vi "Zolix控制 - ZO1.vi"() -> ()   [LabVIEW 2026, in "UI-Zolix.lvlib"]
doc: "本范例执行串口读写操作。串口设置的参数必须匹配连接仪器或设备的参数。“VISA配置串口”VI可设置配置参数。前面板显示的控件可用于配置基本参数，如波特率、数据位和校验。VI会将VISA资源名称传递至其他VI以便执行相关操作。“VISA写入”函数将发送一个命令至串行设备，“VISA读取”函数将返回基于该命令的数据。“VISA关闭”函数可关闭该串行设备的引用。关闭引用十分重要，否则可能导致无法通过该端口进行进一步通信。"
uses:
  UI-Zolix.lvlib
  Supports/Unit.ctl
  Data ColndSave/Supports/Time and Data.ctl
  Supports/Sample Settings.ctl
  Supports/Repeat Steps.ctl
  <userlib>/_NEVSTOP/Communicable State Machine(CSM)/_Polymophic/CSM - Filter Duplicated Lines.vi
  1b2721dc-8cee-4bcb-bbd2-6042867508a2.vi
  b673ad46-ecaf-4cfd-8bbb-6ae2088f5605.vi
  a83f89c7-cc94-454f-8c22-caf8203e03ac.vi
  aa539a88-8cb3-4ee3-9562-2036abd9ba18.vi
  04a4e073-6b30-45d7-bb50-3b2b3a136a6d.vi
  8fd32af9-d1ea-46d4-8c62-5a731f0f3256.vi
  20f4c7ca-4433-4752-8a12-caedff3309a5.vi
  04bf2ced-d956-4811-bd03-133361fc0249.vi
  c4fcee82-142e-4d86-9ec8-28b0cb441057.vi
  2a4e068b-7d24-4fa7-ac03-c345972a0de1.vi
  b1d19f26-e245-4df1-9ac0-43942159cb5b.vi
  6a21441b-8adf-4f54-a790-0ce7b928932a.vi
  796b8098-58f3-468a-8e00-fd722edcd372.vi
  f0ef90a9-37fd-4693-8a17-3839f28c21af.vi
  b45dbba1-636e-4f98-8f9d-e7bac4a6b856.vi
  fd098784-0da8-4741-84dc-d815f177a802.vi
  <userlib>/_NEVSTOP/Communicable State Machine(CSM)/_Polymophic/CSM - Replace Marks in Messages.vi
  990eb54c-669a-44f1-af6b-0d611d3b61bb.vi
  2fc8b641-bc15-4e72-9255-fa26d07ce158.vi
  02d88a95-b21d-42b2-8d64-93e557f2ae07.vi
  4080b3c5-55e2-4fd2-b4b1-a62b83ecccb1.vi
  021cac53-0ee0-419a-8ab1-6e7744cb2707.vi
  72c01e66-041b-423d-8deb-6e79031e249c.vi
  3a72df26-7e5e-43c4-94bb-8d3c34c24f66.vi
  a5163254-29ce-4372-b9a3-2f9bcfab8579.vi
  66bd86cd-02fa-41c1-b7b9-f458bc89fc1e.vi
  6c1f3b6d-07a1-479a-a945-f7a0b01ac58a.vi
  2a40e2d7-c30e-4f84-97eb-49ff59d010fd.vi
  f527ea87-9f16-47b7-892d-a9ab6e0f6a74.vi
  2532b81a-ef6f-4dde-8bfe-c4d2e445e585.vi
  41f7d585-ae95-49ce-8fbc-6366eab20bab.vi
  57b87adc-c73b-462d-8ae1-05c1c70c80b4.vi
  b9a08e84-7226-4261-ac85-d69acd1971d6.vi
  <userlib>/_NEVSTOP/Communicable State Machine(CSM)/AdvanceAPI/CSM - Compact Multiple States.vi
  <userlib>/_NEVSTOP/Communicable State Machine(CSM)/AdvanceAPI/CSM - Break Down Multiple States String.vi
  <userlib>/_NEVSTOP/Communicable State Machine(CSM)/_Shared/Remove Comments from Single-line.vi
  <userlib>/_NEVSTOP/Communicable State Machine(CSM)/_Shared/Split Single-line Message.vi
  <userlib>/_NEVSTOP/Communicable State Machine(CSM)/_Shared/Trim Single-line Text.vi
  <userlib>/_NEVSTOP/Communicable State Machine(CSM)/AdvanceAPI/CSM - Revert Arguments-Safe String.vi
  <userlib>/_NEVSTOP/Communicable State Machine(CSM)/AdvanceAPI/CSM - Make String Arguments Safe.vi
  6a21441b-8adf-4f54-a790-0ce7b928932a.vi/99de0c97-112a-4c86-9094-c187659127e1.vi
  <userlib>/_NEVSTOP/Communicable State Machine(CSM)/Utility/Build Error Cluster.vi
  796b8098-58f3-468a-8e00-fd722edcd372.vi/99de0c97-112a-4c86-9094-c187659127e1.vi
  b45dbba1-636e-4f98-8f9d-e7bac4a6b856.vi/99de0c97-112a-4c86-9094-c187659127e1.vi
  fd098784-0da8-4741-84dc-d815f177a802.vi/99de0c97-112a-4c86-9094-c187659127e1.vi
  2532b81a-ef6f-4dde-8bfe-c4d2e445e585.vi/b09b9099-6be0-413b-8afc-4908471460c3.vi
  <userlib>/_NEVSTOP/Communicable State Machine(CSM)/addons/INI-Static-Variable-Support/_Support/FlagInstance-CSMINIVariable.vi
  b9a08e84-7226-4261-ac85-d69acd1971d6.vi/99de0c97-112a-4c86-9094-c187659127e1.vi
  <vilib>/Utility/error.llb/Trim Whitespace.vi
  <vilib>/Utility/error.llb/Trim Whitespace (string).vi
  <userlib>/_NEVSTOP/Communicable State Machine(CSM)/AdvanceAPI/CSM - Keywords.vi
  <userlib>/_NEVSTOP/Communicable State Machine(CSM)/_Support/ChangeFlag/ChangeFlag-Read.vi
  <vilib>/Utility/error.llb/Trim Whitespace One-Sided.vi
  <userlib>/_NEVSTOP/Communicable State Machine(CSM)/addons/INI-Static-Variable-Support/_Support/instances/_CSM - Read File Logger Configuration - v1.0.vi
  <vilib>/Utility/Data Type/Get Type Information.vi
  <userlib>/_NEVSTOP/Communicable State Machine(CSM)/addons/API-String-Arugments-Support/_Support/Data To SingleElementsArray_csm.vi
  <userlib>/_NEVSTOP/Communicable State Machine(CSM)/addons/API-String-Arugments-Support/_Support/Data To API String Arguments.vi
  <userlib>/_NEVSTOP/Communicable State Machine(CSM)/addons/INI-Static-Variable-Support/_Support/Parse Used Session and Name.vi
  <userlib>/_NEVSTOP/Communicable State Machine(CSM)/addons/INI-Static-Variable-Support/_Support/INI-FGV(lvlibp).vi
  <userlib>/_NEVSTOP/Communicable State Machine(CSM)/addons/INI-Static-Variable-Support/_Support/Populate String with INI Variable.vi
  <userlib>/_NEVSTOP/Communicable State Machine(CSM)/addons/API-String-Arugments-Support/_Support/Convert API String Arguments to Data(variant).vi
  <userlib>/_NEVSTOP/Communicable State Machine(CSM)/addons/API-String-Arugments-Support/_Support/SingleElementsArray To Data_csm.vi
  <userlib>/_NEVSTOP/Communicable State Machine(CSM)/addons/MassData-Parameter/_support/FGV-MassData(lvlibp).vi
  <vilib>/Instr/_visa.llb/VISA Configure Serial Port (Instr).vi
  Repeat/Repeat.vi
  <userlib>/_NEVSTOP/Communicable State Machine(CSM)/_Support/ChangeFlag/ChangeFlagDB.vi
  <userlib>/_NEVSTOP/Communicable State Machine(CSM)/Communicable State Machine.lvlib
  Data ColndSave/Data Collection and Save.lvlib
  <userlib>/_NEVSTOP/Communicable State Machine(CSM)/addons/INI-Static-Variable-Support/INI-Static-Variable-Support.lvlib
  <userlib>/_NEVSTOP/Communicable State Machine(CSM)/addons/MassData-Parameter/CSM MassData Parameter Support.lvlib
  <userlib>/_NEVSTOP/Communicable State Machine(CSM)/addons/Watchdog/CSM Watchdog.lvlib
  <userlib>/_NEVSTOP/Communicable State Machine(CSM)/addons/Logger/CSM File Logger.lvlib
  Logging/Logging.lvlib
  Acquisition/Acquisition.lvlib
  Repeat/Repeat.lvlib
panel:
  out "Current Position":dbl
  in  "停止":bool
  in  "Zolix显示":enum32{"Zolix控制", "循环功能", "联动功能", "Status"}(tab)
  out "Zolix电机位置":waveform(dbl)(graph)
  in  "USB Port":refnum<visa-resource-name>
  in  "CSM Name":string="ZO1"
  in  "归零速度":dbl=10.0
  in  "初速度":dbl=10.0
  in  "加速度":dbl=10.0
  in  "常速度":dbl=10.0
  out "运行中？":bool
  in  "位置坐标1":dbl=10.0
  in  "位置1":bool
  out "当前坐标 T":dbl format="%#.2f"
  out "当前坐标 Z":dbl format="%#.2f"
  out "当前坐标 Y":dbl format="%#.2f"
  out "当前坐标X":dbl format="%#.2f"
  in  "用户原点归零":bool
  in  "光学归零":bool
  in  "负限位归零":bool
  in  "连续前进":bool
  in  "连续后退":bool
  in  "位置坐标2":dbl=10.0
  in  "单位":T1
  in  "位置2":bool
  in  "运动距离":sgl=10.0
  in  "后退":bool
  in  "前进":bool
  in  "Zolix停止":bool
  in  "坐标选择":enum32{"X", "Y", "Z", "T"}(radio)
  out "状态信息":string
  in  "Zolix_USB连接":bool
  in  "Interval(s)":dbl=0.5
  in  "Zolix循环功能":bool
  out "State History":string
  out "Error Occurred":errorcluster caption="Zolix-错误输出"
  in  "子程序？":bool
  # "相对位移"
  # "绝对位移"
  # "连续移动"
  # "归零"
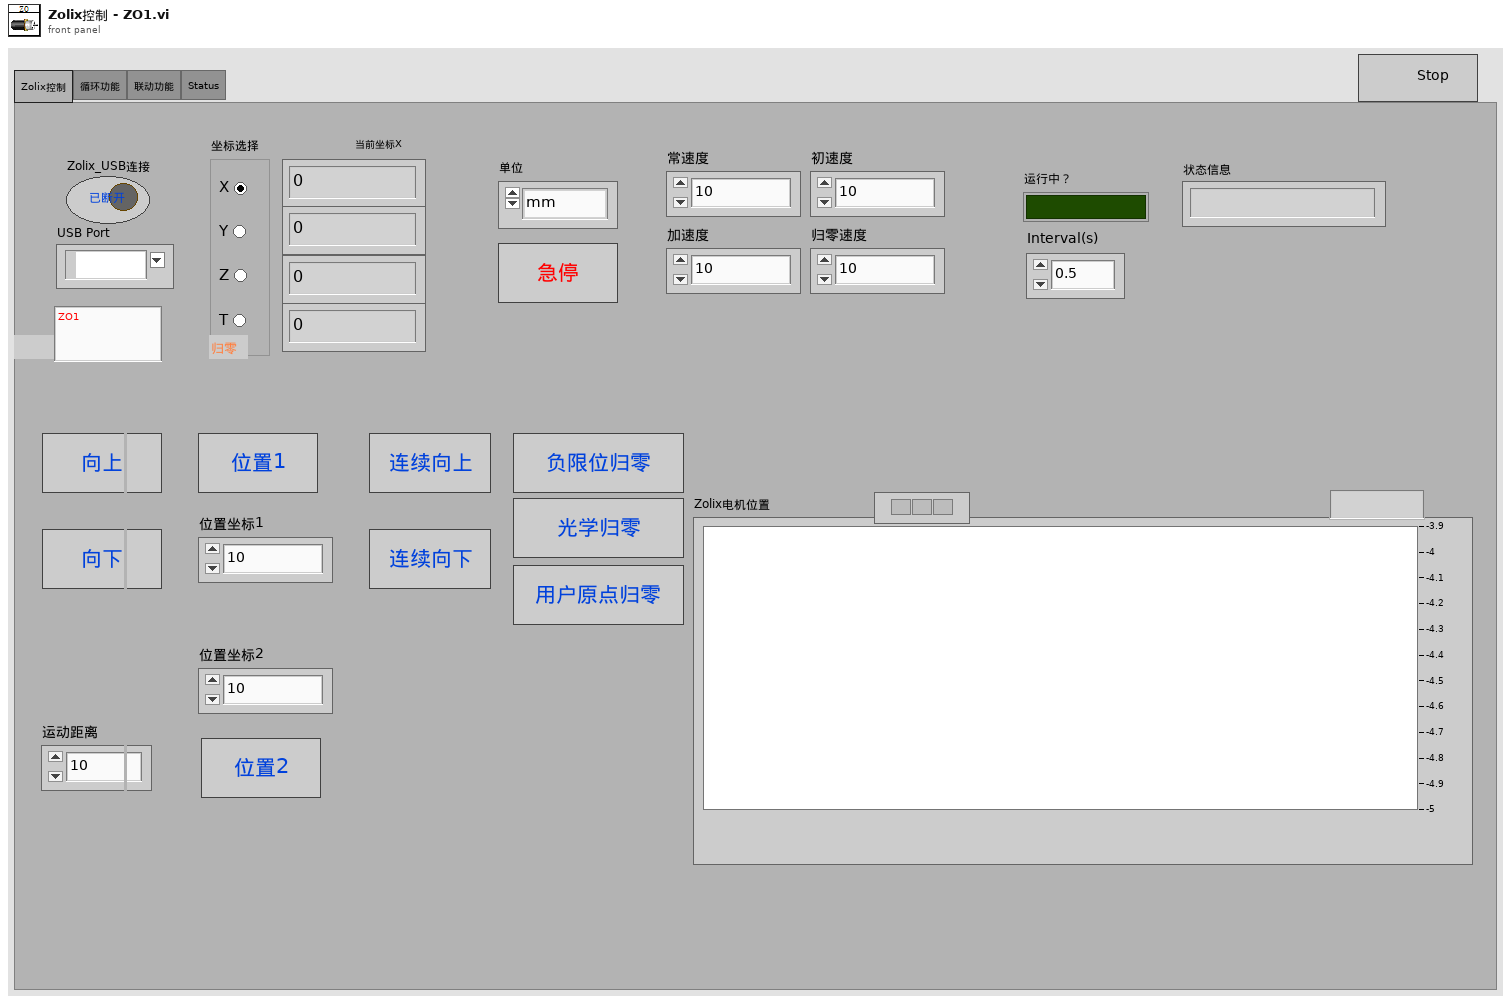
[diagram p1: front panel]
types:
  T1 = typedef "UI-Zolix.lvlib/Unit.ctl" = enum16{"mm", "um", "PP", "deg"}
  T2 = cluster{"Enable":bool, "Limit":cluster{"FileSize":i64, "FileNum":i32}, "Timestamp.Format":string, "AutoExit":bool}
  T3 = enum32{"Invalid", "Standard", "Closed", "Hidden", "Minimized", "Maximized"}
  T4 = enum32{"invalid app kind", "Development System", "Run Time System", "Student Edition", "Embedded LabVIEW", "Evaluation", "Custom"}
  T5 = enum8{"Enabled", "Disabled", "Disabled and Grayed Out"}
  T6 = cluster{"波特率":u32, "数据位":u16, "校验":enum16{"None", "Odd", "Even", "Mark", "Space"}, "停止位":u16, "流控制":u16}
  T7 = typedef "Communicable State Machine.lvlib/_CSM_Response Source Message.ctl" = cluster{"‘State":string, "’Arguments":string, "’Error":errorcluster}
  T8 = cluster{"Current VI Reference":refnum<vi>, "Close Panel on Exit?":bool}
  T9 = typedef "UI-Zolix.lvlib/Sample Settings.ctl" = cluster{"USB Port":refnum<visa-resource-name>, "采集间隔(s)":dbl, "坐标选择":enum32{"X", "Y", "Z", "T"}, "Axis":string[], "Unit":string[]}
  T10 = typedef "Data Collection and Save.lvlib/Time and Data.ctl" = cluster{"采集时间":timestamp, "Data":dbl[]}
  T11 = cluster{"Core":cluster{"Current VI Reference":refnum<vi>, "Close Panel on Exit?":bool}, "Device Info":T9, "Time and Data":T10, "子程序？":bool, "Device Status":cluster{"常速度":dbl, "初速度":dbl, "归零速度":dbl, "加速度":dbl, "运动距离":dbl, "单位":T1}}
  T12 = cluster{"常速度":dbl, "初速度":dbl, "归零速度":dbl, "加速度":dbl, "运动距离":dbl, "单位":T1}
  T13 = typedef "UI-Zolix.lvlib/Repeat Steps.ctl" = cluster{"行程":dbl, "时间(s)":dbl, "进度":dbl, "光谱测量拿起":bool, "运行方向":bool, "速度":dbl, "分段颜色":enum32{"蓝色", "红色"}}[]
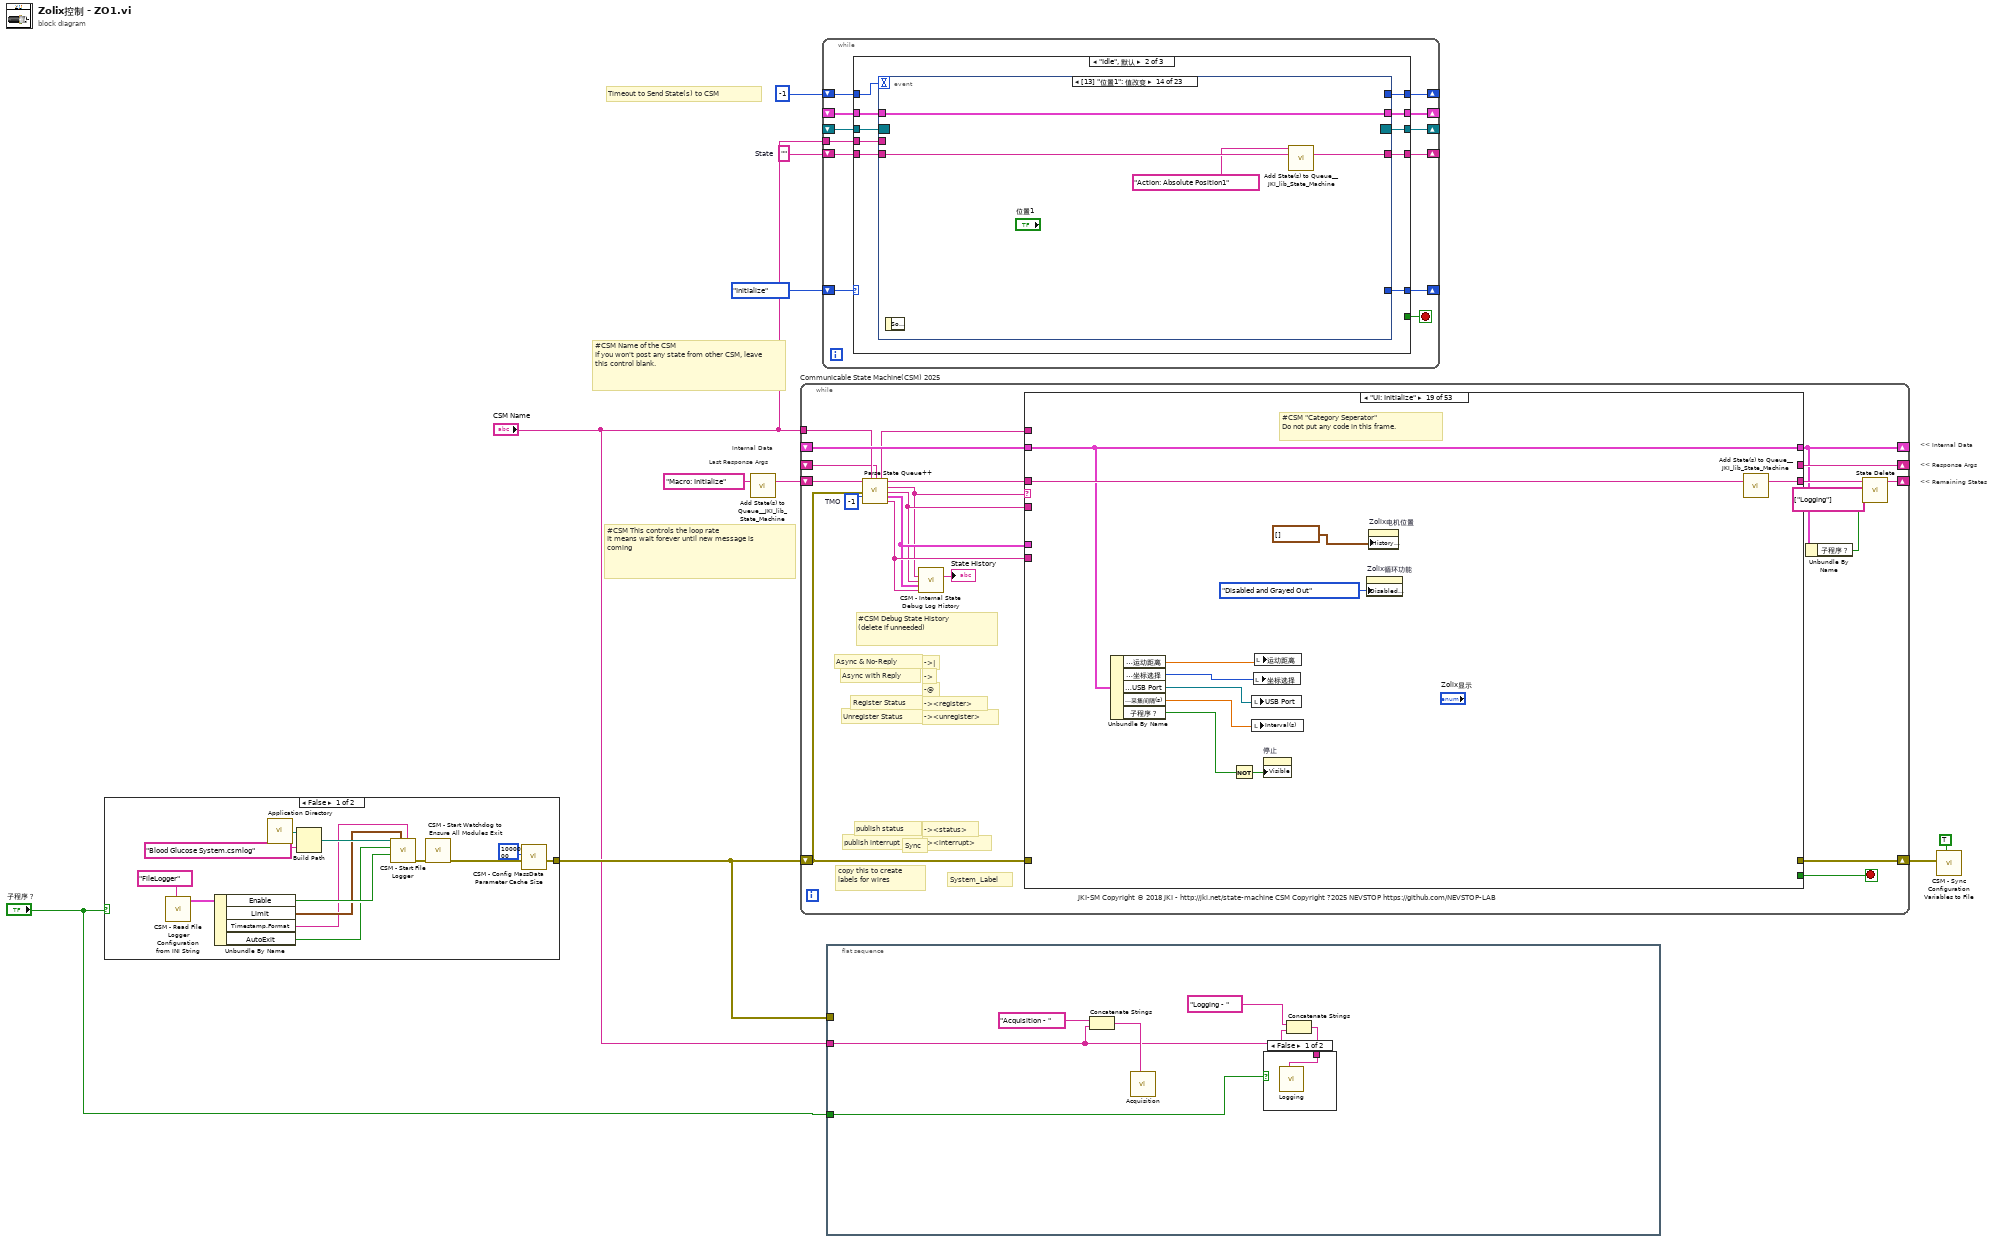
[diagram p0: block diagram]
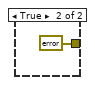
[diagram p2: hidden frame]
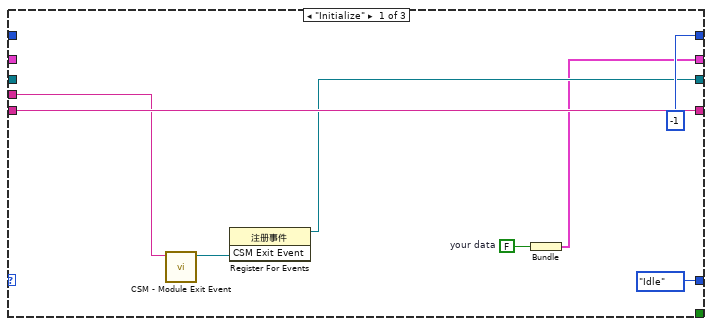
[diagram p4: hidden frame]
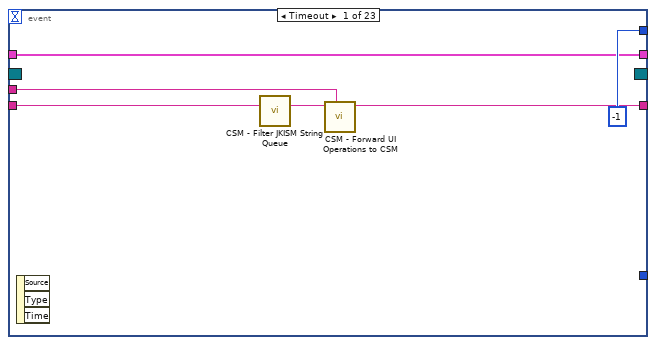
[diagram p5: hidden frame]
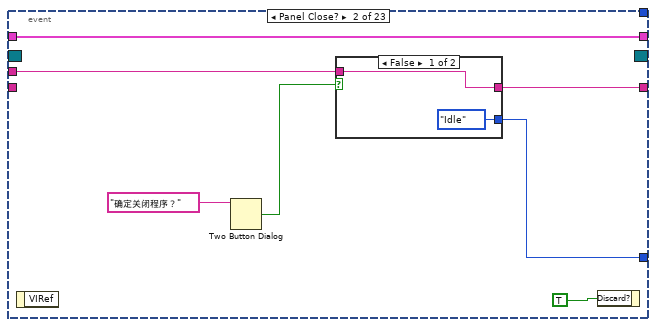
[diagram p6: hidden frame]
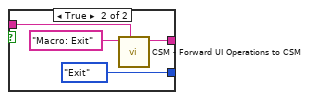
[diagram p7: hidden frame]
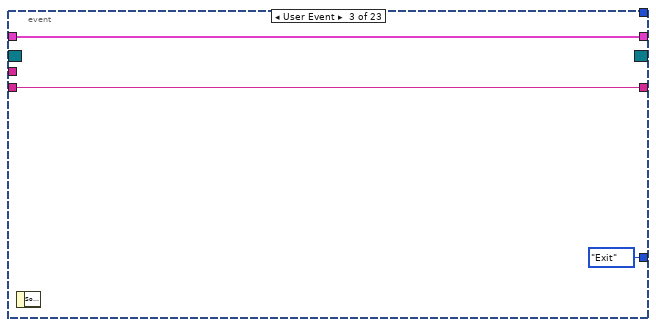
[diagram p8: hidden frame]
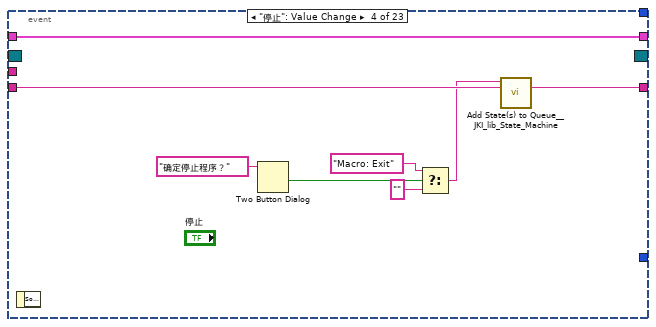
[diagram p9: hidden frame]
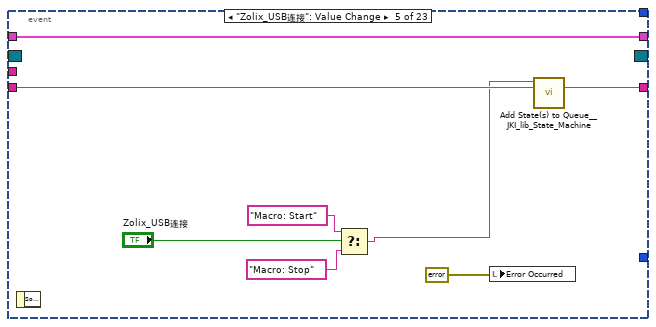
[diagram p10: hidden frame]
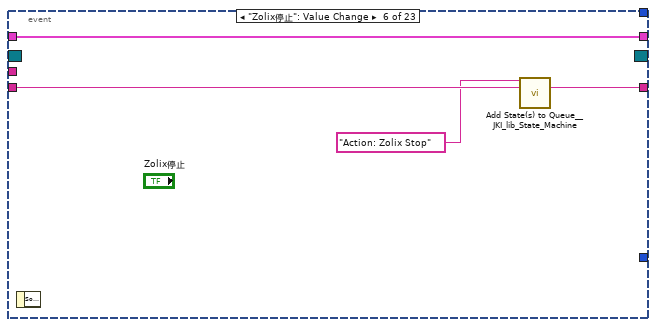
[diagram p11: hidden frame]
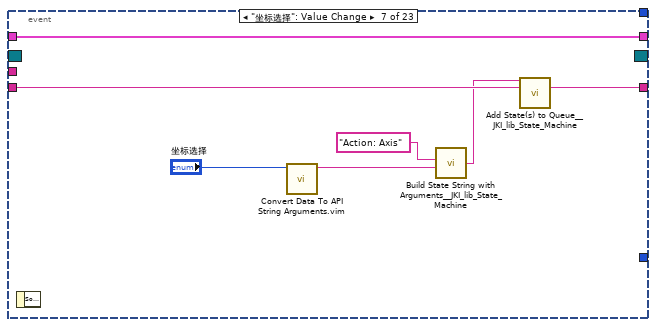
[diagram p12: hidden frame]
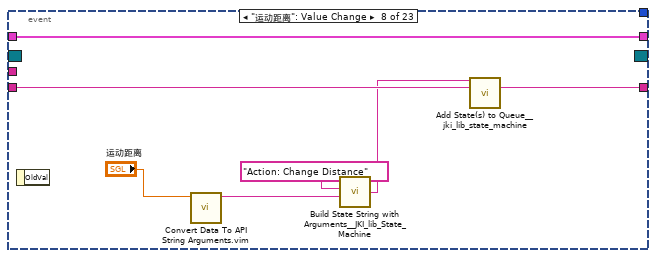
[diagram p13: hidden frame]
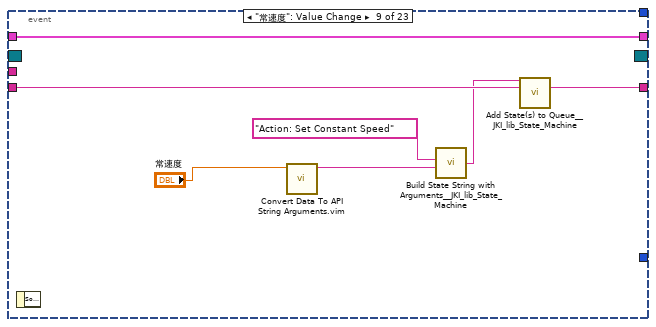
[diagram p14: hidden frame]
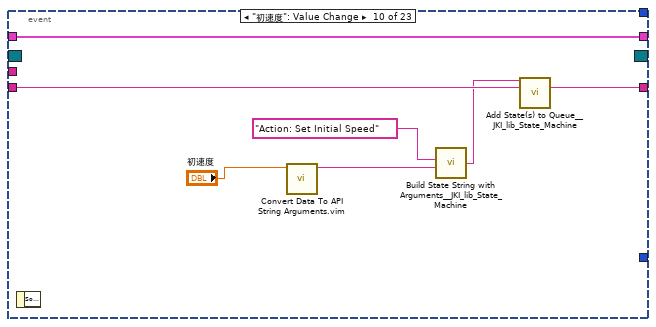
[diagram p15: hidden frame]
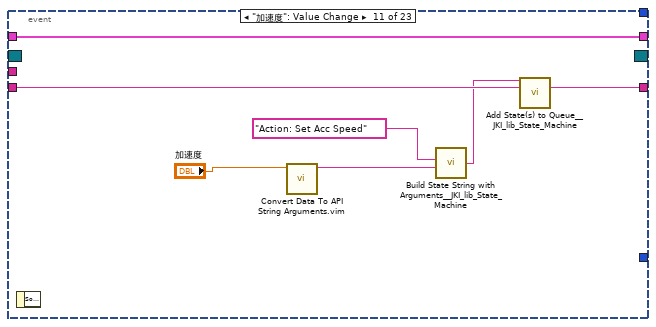
[diagram p16: hidden frame]
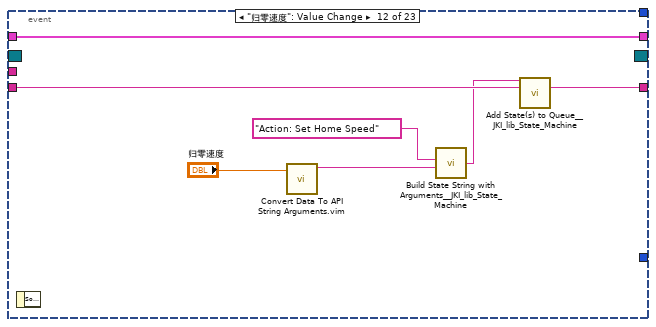
[diagram p17: hidden frame]
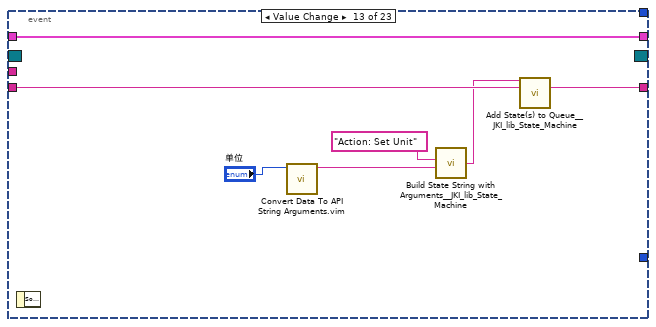
[diagram p18: hidden frame]
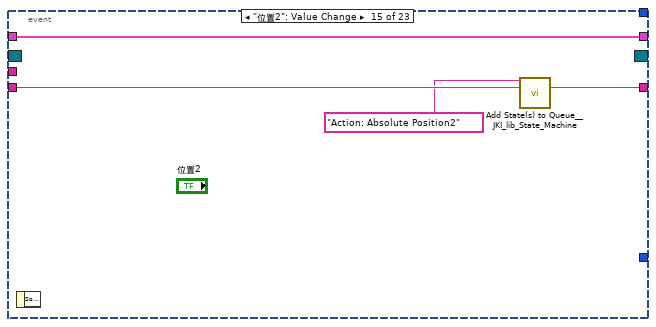
[diagram p19: hidden frame]
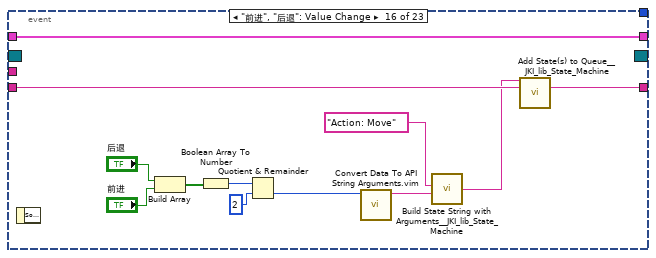
[diagram p20: hidden frame]
diagram:
  w9 = ""  # State
  # "Timeout to Send State(s) to CSM"
  # "Last Response Args"
  # "Internal Data"
  # "#CSM Name of the CSM\nIf you won't post any state from other CSM, leave this control blank."
  # "#CSM This controls the loop rate\nIt means wait forever until new message is coming"
  # "<< Internal Data"
  # "<< Response Args"
  # "<< Remaining States"
  n1 = case shown="False" "子程序？" {
    tunnel: [w11 errorcluster {"status"=FALSE, "code"=0, "source"=""} ("Error out")] -> w5
    frame False {
      n2 = call-poly <userlib>:"CSM - Read File Logger Configuration from INI String.vi"("Section Name(\"FileLogger\")"="FileLogger" ("Section Name(\"\" as Default)")) -> ("FileLogger Configuration-v1"=w18:T2)  [unwired: 7 in, 1 out]
      n3 = Unbundle By Name(w18) -> ("Enable"=w17:bool, "Limit"=w16:cluster{"FileSize":i64, "FileNum":i32}, "Timestamp.Format"=w14:string, "AutoExit"=w15:bool)
      n4 = call <vilib>:"Application Directory.vi"() -> ("Application Directory"=w23:path)
      n5 = Build Path(base path=w23, name or relative path="Blood Glucose System.csmlog") -> (appended path=w21:path)
      n6 = call <userlib>:"CSM - Start File Logger.vi"("Timestamp Format"=w14, "Log Limit"=w16, "Watchdog? (T)"=w17, "Exit When All Module Exist? (F)"=w15, "Log File Path"=w21) -> ("error out"=w20:errorcluster)  [unwired: 4 in, 2 out]
      n7 = call <userlib>:"CSM - Start Watchdog to Ensure All Modules Exit.vi"("error in (no error)"=w20) -> ("error out"=w12:errorcluster)  [unwired: 10 in]
      n8 = call <userlib>:"CSM - Config MassData Parameter Cache Size.vi"("Error in"=w12, "Size (50M)"=1000000 ("size(1M)")) -> ("Error out"=w11:errorcluster)  [unwired: 9 in]
    }
    frame True {
    }
  }
  n9 = call <vilib>:"Add State(s) to Queue__JKI_lib_State_Machine.vi"("State(s) in (\"\")"="Macro: Initialize" ("Init State(\"Macro: Initialize\")")) -> ("States Out"=w6:string)  [unwired: 14 in]
  n10 = while "Communicable State Machine(CSM) 2025" {
    shift-right: [w26] -> _
    shift-left: _ -> [w41]
    shift-right: [w43] -> w3
    shift-left: w5 -> [w31]
    shift-right: [w28] -> _
    shift-left: w6 -> [w44]
    tunnel: "CSM Name" -> [w38]
    shift-right: [w39] -> _
    shift-left: _ -> [w33]
    stop <- w42 stop-if-true
    w40 = -1  # TMO
    # "#CSM Debug State History\n(delete if unneeded)"
    # "-><interrupt>"
    # "-><status>"
    # "-><unregister>"
    # "-><register>"
    # "-@"
    # "->"
    # "->|"
    # "publish interrupt"
    # "publish status"
    # "Unregister Status"
    # "Register Status"
    # "Sync"
    # "Async with Reply"
    # "Async & No-Reply"
    # "JKI-SM Copyright © 2018 JKI - http://jki.net/state-machine CSM Copyright ?2025 NEVSTOP https://github.com/NEVSTOP-LAB"
    # "copy this to create labels for wires"
    # "System_Label"
    n11 = call <userlib>:"Parse State Queue++.vi"("State Queue"=w44, "Name (\"\" to Use UUID)"=w38, "Response Arguments"=w33, "Previous Error"=w31, "Dequeue (1 ms)"=w40) -> ("Name Used"=w32:string, "Remaining States"=w45:string, "Current State"=w34:string, "Arguments"=w35:string, "Additional Information"=w36:T7, "Source CSM"=w37:string)  [unwired: 5 in]
    n12 = call <userlib>:"CSM - Internal State Debug Log History.vi"("State"=w34, "Arguments (\"\")"=w35, ">> Response Source Message >>"=w36, "Source (\"\")"=w37) -> ("Debug Log"=→"State History":string)  [unwired: 11 in]
    n13 = case shown="\"UI: Initialize\"" w34 {
      selector: w34 -> [_ _ _ w56 _ _ _ _ _ _ _ _ _ _ _ _ _ _ _ _ _ _ _ _ _ _ _ _ _ _ _ _ _ _ _ _ _ _ _ _ _ _ _ _ _ _ _ _ _ _ _ _ _]
      tunnel: w45 -> [w46 w49 w52 w60 w65 w71 w96 w102 w108 w118 w125 w137 w141 w144 w162 w176 w192 w195 w206 w217 w220 w226 w252 w260 w267 w273 w274 w277 w288 w296 w303 w323 w335 w366 w381 w397 w413 w429 w447 w471 w495 w513 w530 w545 w561 w564 w575 w582 w584 w598 w614 w623 w630]
      tunnel: w35 -> [_ _ _ _ _ w70 w92 w99 w105 w112 _ _ _ _ _ w174 _ _ _ _ _ _ _ _ _ _ _ _ _ w295 w302 w322 _ _ w379 w385 w401 w417 _ _ w494 w498 _ _ _ _ w569 w580 _ _ w611 _ _]
      tunnel: w41 -> [w47 w48 w50 w58 w64 w76 w94 w100 w106 w116 w124 w131 w139 w142 _ w165 w187 w193 w196 w215 w218 w224 w250 w255 w265 w271 w276 w279 w287 w293 w299 w320 w334 w365 w380 w386 w402 w418 w449 w454 w478 w499 w529 w532 w548 w566 w568 w579 w586 w600 w616 w625 w632]
      tunnel: [_ _ _ w53 w66 errorcluster {"status"=FALSE, "code"=0, "source"=""} ("error out") w89 w97 w103 w119 _ _ _ _ _ _ w188 _ _ _ _ _ w229 _ w262 _ _ _ _ _ w305 w316 w337 w342 w383 w399 w415 w431 w451 w470 w497 w515 w519 w547 w563 _ _ _ w587 w601 w617 w626 w633] -> w43
      tunnel: w31 -> [_ _ _ w54 w66 w74 w90 w98 w104 _ _ _ _ _ _ _ w189 _ _ _ _ _ _ _ w263 _ _ _ w285 _ w305 w317 w337 _ w383 w399 w415 w431 w451 _ w497 w515 _ w547 w563 _ _ _ w587 w601 w617 w626 w633]
      tunnel: [w46 w49 w51 w59 w65 w72 w95 w101 w107 w117 w125 w136 w140 w143 w161 w175 w191 w194 w205 w216 w219 w225 w251 w259 w267 w272 w275 w278 w289 w297 w304 w324 w336 w367 w382 w398 w414 w430 w448 w472 w496 w514 w531 w546 w562 w565 w576 w583 w585 w599 w615 w624 w631] -> w29
      tunnel: [_ _ _ _ _ _ TRUE _ _ _ _ _ TRUE _ _ _ _ _ _ _ _ _ _ _ _ _ _ _ _ _ _ _ _ _ _ _ _ _ _ _ _ _ _ _ _ _ _ _ _ _ _ _ _] -> w42
      tunnel: [w47 w48 w50 w58 w64 w76 w94 w100 w106 w115 w124 w135 w139 w142 w160 w164 w187 w193 w196 w215 w218 w224 w242 w255 w265 w271 w276 w279 w287 w291 w298 w321 w332 w365 w380 w386 w402 w418 w449 w454 w478 w499 w529 w532 w548 w566 w567 w578 w586 w600 w616 w625 w632] -> w26
      tunnel: w37 -> [_ _ _ _ _ w69 _ _ _ w113 _ _ _ _ _ _ _ _ _ _ _ _ _ _ _ _ _ _ _ _ _ _ _ _ _ _ _ _ _ _ _ _ _ _ _ _ _ _ _ _ _ _ _]
      tunnel: w36 -> [_ _ _ _ _ w68 _ _ _ w114 _ _ _ _ _ _ _ _ _ _ _ _ _ _ _ _ _ _ _ _ _ _ _ _ _ _ _ _ _ _ _ _ _ _ _ _ _ _ _ _ _ _ _]
      tunnel: [_ _ _ "" w61 _ _ _ _ _ _ _ _ _ _ _ _ _ _ _ _ _ _ _ _ _ _ _ _ _ _ _ _ _ _ _ _ _ _ _ _ _ _ _ _ _ _ _ _ _ _ _ _] -> w39
      tunnel: w32 -> [_ _ _ w55 _ _ w91 _ _ _ _ _ _ _ w146 _ w183 _ _ _ _ w222 w247 w257 _ w269 _ _ _ _ _ _ _ _ _ _ _ _ _ _ _ _ _ _ _ _ w573 _ _ w590 w610 _ _]
      frame "", "Idle" {
        # "#CSM \"Idle/Event Handler\"\nexecutes when the state queue is empty"
      }
      frame "CSM Documentation" {
        # "#CSM State Syntax\n\n// Comment line, all text to the right of “//” will be ignored\n// Local Message Example\nDoSth: DoA >> Arguments\n\n// Sync Call Example\nAPI: xxxx >> Arguments -@ TargetModule\n\n// Async Call Example\nAPI: xxxx >> Arguments -> TargetModule\n\n// Async Call without Reply Example\nAPI: xxxx >> Arguments ->| TargetModule\n\n// Broadcast normal status:\nStatus >> StatusArguments  -><status>\n\n// Broadcast Interrupt status:\nInterrupt >> StatusArguments  -><interrupt>\n\n// Register Source Module's status to Handler Module\nStatus@Source Module >> Handler Module@Handler Module -><register>\n\n// Unegister Source Module's status\nStatus@Source Module >> Handler Module -><unregister>"
        # "#CSM README FIRST\n\nCommunicable State Machine(CSM) is a LabVIEW application framework that builds upon JKI State Machine(JKISM). It follows the pattern of JKISM and extends the keywords to describe message communication between modules, including concepts such as Sync-Message, Async-Message, Subscription/Unsubscription of status - essential elements for creating reusable code modules. For more information, please visit the CSM wiki: https://nevstop-lab.github.io/CSM-Wiki/\n\nFor instructions on JKI State Machine, visit: \n    http://jki.net/state-machine/\nFor information about CSM, visit: \n    https://github.com/NEVSTOP-LAB"
        # "#CSM \"Documentation\"\nCase for holding CSM Documenation"
      }
      frame "---------- Core ----------" {
        # "#CSM \"Category Seperator\"\nDo not put any code in this frame."
        n14 = call <vilib>:"Add State(s) to Queue__JKI_lib_State_Machine.vi"("State(s) in (\"\")"=w52) -> ("States Out"=w51:string)  [unwired: 14 in]
      }
      frame Default {
        # "#CSM \"Default\"\nthis is used to capture unhandled states and typos"
        n15 = call <userlib>:"CSM Unhandled State Error.vi"("error in (no error)"=w54, "Undefined State"=w56, "CSM Name"=w55) -> ("error out"=w53:errorcluster)  [unwired: 8 in]
        n16 = call <vilib>:"Add State(s) to Queue__JKI_lib_State_Machine.vi"("State(s) in (\"\")"=w60) -> ("States Out"=w59:string)  [unwired: 14 in]
      }
      frame "VI Reference" {
        n17 = Unbundle By Name(w64) -> ("Core"=w63:T8)
        n18 = Unbundle By Name(w63) -> ("Current VI Reference"=w62:refnum<vi>)
        n19 = call <userlib>:"CSM - Convert Data to HexStr.vi"("Variant"=w62) -> ("HEX String (0-9,A-F)"=w61:string)  [unwired: 8 in]
      }
      frame "Error Handler" {
        # "#CSM \"Error Handler\"\nYou can also output any states to clean-up after errors occur"
        # "Clear error"
        n20 = case shown="错误" w74 {
          selector: w74 -> [_ w83]
          tunnel: [w81 w85] -> w73
          tunnel: w71 -> [w81 w84]
          tunnel: w70 -> [w80 _]
          tunnel: w69 -> [_ _]
          tunnel: w68 -> [_ _]
          tunnel: [w78 w83] -> w67
          frame No Error {
            n21 = call <userlib>:"CSM - Convert Argument to Error.vi"("Argument"=w80) -> ("Error"=w79:errorcluster)  [unwired: 4 in]
            n22 = flat-sequence {
              tunnel: w79 -> [w82]
              tunnel: [w82] -> w78
              frame #0 {
              }
            }
          }
          frame Error {
            # "#CSM Internal Error Handler Case \nIf any error Occurred, \"Error Occurred\" \nstatus update will be broadcasted to system.\nParameter is Error Cluster."
            n23 = call <userlib>:"CSM - Convert Error to Argument.vi"("Error"=w83) -> ("Argument"=w87:string)  [unwired: 4 in]
            n24 = call <vilib>:"Build State String with Arguments__JKI_lib_State_Machine.vi"("Arguments (\"\")"=w87, "State"="Error Occurred" ("Status with Arguments")) -> ("State with Arguments"=w86:string)  [unwired: 4 in]
            n25 = call <userlib>:"CSM - Broadcast Status Change.vi"("Status With Arguments"=w86, "State Queue"=w84) -> ("Remaining States"=w85:string)  [unwired: 13 in]
          }
        }
        "Error Occurred" <- w67
        n26 = call <vilib>:"Add State(s) to Queue__JKI_lib_State_Machine.vi"("State(s) in Front (\"\")"="// Post Error States", "State(s) in (\"\")"=w73) -> ("States Out"=w72:string)  [unwired: 13 in]
      }
      frame "Critical Error" {
        # "#CSM \"Critical Error\"\nWhen any un-recoverable error occurs, CSM goes into this case."
        # "#CSM Stop in Critical Error\nWhen Critical Error occurs, Stop the loop immediately. Do NOT change this unless you fully understand the impact."
        n27 = call <userlib>:"CSM Critical Error.vi"("error in (no error)"=w90, "Arugments (As Reason)"=w92, "CSM Name"=w91) -> ("error out"=w89:errorcluster)  [unwired: 8 in]
        n28 = call <vilib>:"Add State(s) to Queue__JKI_lib_State_Machine.vi"("State(s) in (\"\")"=w96) -> ("States Out"=w95:string)  [unwired: 14 in]
      }
      frame "Target Timeout Error" {
        # "#CSM \"Target Timeout Error\"\nWhen This CSM could not get the sync-call response in time, This CSM goes into this case."
        n29 = call <userlib>:"CSM Target Timeout Error.vi"("error in (no error)"=w98, "Arguments (As CSM Name)"=w99) -> ("error out"=w97:errorcluster)  [unwired: 9 in]
        n30 = call <vilib>:"Add State(s) to Queue__JKI_lib_State_Machine.vi"("State(s) in (\"\")"=w102) -> ("States Out"=w101:string)  [unwired: 14 in]
      }
      frame "Target Error" {
        # "#CSM \"Target Error\"\nWhen This CSM try to communicate with an un-existed CSM, This CSM goes into this case."
        n31 = call <userlib>:"CSM Target Error.vi"("error in (no error)"=w104, "Arguments (As CSM Name)"=w105) -> ("error out"=w103:errorcluster)  [unwired: 9 in]
        n32 = call <vilib>:"Add State(s) to Queue__JKI_lib_State_Machine.vi"("State(s) in (\"\")"=w108) -> ("States Out"=w107:string)  [unwired: 14 in]
      }
      frame "Async Response", "Response" {
        n33 = Unbundle(w114) -> ("‘State"=w111:string, "’Arguments"=w110:string, "’Error"=w109:errorcluster)
        n34 = case shown="默认" w111 {
          tunnel: [w120] -> w117
          tunnel: w118 -> [w121]
          tunnel: [w123] -> w115
          tunnel: w116 -> [w123]
          tunnel: [w122] -> w119
          tunnel: w109 -> [w122]
          tunnel: w113 -> [_]
          tunnel: w112 -> [_]
          tunnel: w110 -> [_]
          frame 默认 {
            # "#CSM \"Async Response\"\nHandle Async-call Response (\"Async Response\" for ->)"
            # "#CSM \"Response\"\nHandle Sync-call Response (\"Response\" for -@)"
            # "#CSM Response Comments\nAfter Message is executed, CSM goes to this state for receive the response.\n    For Async Message(->), \"Async Response\" is used. This CSM will goes to \"Async Message Posted\" immediately and receive the \"Async Response\" after the callee finishes the message.\n    For Sync Message(@),  This CSM will wait until the message is done and immediately goes to \"Response\""
            n35 = call <vilib>:"Add State(s) to Queue__JKI_lib_State_Machine.vi"("State(s) in (\"\")"=w121) -> ("States Out"=w120:string)  [unwired: 14 in]
          }
        }
      }
      frame "Async Message Posted" {
        # "#CSM \"Async Message Posted\"\nAfter Async Message is posted (-> or ->| ), CSM goes to this state for post-action.\nYou can use Argument - State to tell which Async Message is called."
      }
      frame "Initialize Core Data" {
        # "#CSM \"Initialize Core Data\"\nThis is used to determine panel behavior on exit"
        # "originally closed?"
        # "exe?"
        # "If panel starts closed or is an EXE, then close it when we exit"
        n36 = property class="VI"() -> ("FP.State"=w128:T3)  [unwired: 2 in, 2 out]
        n37 = property class="App"() -> ("App.Kind"=w134:T4)  [unwired: 2 in, 2 out]
        n38 = control-ref of="Current VI Reference"() -> (w129:refnum<vi>)
        n39 = Equal?(x=w128, y=T3."Closed" ("Front Panel Window:State")) -> (x = y?=w126:bool)
        n40 = Equal?(x=w134, y=T4."Run Time System" ("Application:Kind")) -> (x = y?=w132:bool)
        n41 = Or(x=w126, y=w132) -> (x .or. y?=w130:bool)
        n42 = Bundle By Name(cluster=w131, "Core.Current VI Reference"=w129, "Core.Close Panel on Exit?"=w130) -> (w135:T11)
        n43 = call <vilib>:"Add State(s) to Queue__JKI_lib_State_Machine.vi"("State(s) in (\"\")"=w137) -> ("States Out"=w136:string)  [unwired: 14 in]
      }
      frame "Exit" {
        # "#CSM \"Exit\"\nCase for exiting the loop. No errors that occur here will be handled."
        n44 = call <vilib>:"Add State(s) to Queue__JKI_lib_State_Machine.vi"("State(s) in (\"\")"=w141) -> ("States Out"=w140:string)  [unwired: 14 in]
      }
      frame "---------- Data ----------" {
        # "#CSM \"Category Seperator\"\nDo not put any code in this frame."
        n45 = call <vilib>:"Add State(s) to Queue__JKI_lib_State_Machine.vi"("State(s) in (\"\")"=w144) -> ("States Out"=w143:string)  [unwired: 14 in]
      }
      frame "Data: Initialize" {
        w147 = T12 {"常速度"=10.0, "初速度"=10.0, "归零速度"=10.0, "加速度"=10.0, "运动距离"=10.0, "单位"=enum."mm"}  # Device Status
        w151 = T9 {"USB Port"="", "采集间隔(s)"=0.5, "坐标选择"=enum."X", "Axis"=["X", "Y", "Z", "T"], "Unit"=["m", "u", "s", "d"]}  # Device Info
        w150 = FALSE ("结束")
        w157 = T10 {"采集时间"=timestamp(0 s since 1904-01-01), "Data"=[0.0, 0.0]}  # Time and Data
        w159 = T8 {"Current VI Reference"=refnum, "Close Panel on Exit?"=FALSE}  # Core
        # "#CSM \"Data: Initialize\"\nInitialize the shift-register data, here.\n(data names are defined by what you wire into the bundle function)"
        # "#CSM do not delete - used by framework"
        # "#CSM Data names and types of shift register data are defined by this bundle."
        n46 = local write "Error Occurred"(errorcluster {"status"=FALSE, "code"=0, "source"=""} ("Error Occurred")) -> ()
        n47 = local read "子程序？"() -> (w156:bool)
        n48 = call "CSM - Read Cluster Elements From Session.vim"("Section Name (\"\" as Default)"=w146, "Cluster"=w151) -> ("Cluster out"=w155:T9)  [unwired: 6 in, 1 out]
        n49 = local write "Zolix_USB连接"(w150) -> ()
        n50 = call "CSM - Read Cluster Elements From Session.vim"("Section Name (\"\" as Default)"=w146, "Cluster"=w147) -> ("Cluster out"=w149:T12)  [unwired: 6 in, 1 out]
        n51 = local write "Zolix循环功能"(w150) -> ()
        n52 = Select(t=w155, s=TRUE, f=w151) -> (s? t:f=w153:T9)
        n53 = Select(t=w149, s=TRUE, f=w147) -> (s? t:f=w145:T12)
        n54 = Bundle("Core"=w159, "Device Info"=w153, "Time and Data"=w157, "子程序？"=w156, "Device Status"=w145) -> (w160:T11)  [unwired: 1 in]
        n55 = call <vilib>:"Add State(s) to Queue__JKI_lib_State_Machine.vi"("State(s) in (\"\")"=w162) -> ("States Out"=w161:string)  [unwired: 14 in]
        "状态信息" <- "" ("状态信息")
      }
      frame "Data: Update Indicators" {
        w173 = T10 {"采集时间"=timestamp(0 s since 1904-01-01), "Data"=[]}  # Time and Data
        n56 = call "CSM - Convert Argument to MassData.vim"("Type"=w173, "MassData Argument"=w174) -> ("Data"=w163:T10)  [unwired: 6 in, 1 out]
        n57 = Unbundle By Name(w165) -> ("Device Info.坐标选择"=w170:enum32{"X", "Y", "Z", "T"})
        n58 = Unbundle By Name(w163) -> ("Data"=w172:dbl[])
        n59 = Index Array(array=w172) -> (element=w171:dbl)  [unwired: 1 in]
        n60 = case shown="\"X\", 默认" w170 {
          tunnel: w171 -> [w179 w180 w181 w182]
          tunnel: [w179 w180 w181 w182] -> w167
          frame "X", Default {
            "当前坐标X" <- w179
          }
          frame "Y" {
            "当前坐标 Y" <- w180
          }
          frame "Z" {
            "当前坐标 Z" <- w181
          }
          frame "T" {
            "当前坐标 T" <- w182
          }
        }
        "Current Position" <- w167
        n61 = in-place {
          in-place-border: w163 -> [w178]
          n62 = in-place-cluster #1(w165) -> ()  [unwired: 1 out]
          n63 = in-place-cluster #1("Time and Data"=w178) -> (w164:T11)
        }
        n64 = feedback #2 ("反馈节点")(0.0 ("GetPosition")) -> (w168:dbl)
        n65 = feedback-in #2(w167) -> ()
        n66 = Not Equal?(x=w168, y=w167) -> (x != y?=→"运行中？":bool)
        n67 = call <vilib>:"Add State(s) to Queue__JKI_lib_State_Machine.vi"("State(s) in Front (\"\")"="UI: Update Graph" ("State(s) in Front (\"\")"), "State(s) in (\"\")"=w176) -> ("States Out"=w175:string)  [unwired: 13 in]
      }
      frame "Data: Cleanup" {
        # "#CSM \"Data: Cleanup\"\nCleanup any data and references, here.\n(this is called automatically, by the Macro: Exit)"
        n68 = Unbundle By Name(w187) -> ("Core.Current VI Reference"=w190:refnum<vi>, "Device Info"=w186:T9, "Device Status"=w184:T12)
        n69 = call "CSM - Write Configuration Variable.vim"("Section Name (\"\" as Default)"=w183, "Configuration"=w186) -> ()  [unwired: 6 in, 2 out]
        n70 = call "CSM - Write Configuration Variable.vim"("Section Name (\"\" as Default)"=w183, "Configuration"=w184) -> ()  [unwired: 6 in, 2 out]
        n71 = Close Reference(reference=w190, error in (no error)=w189) -> (error out=w188:errorcluster)
        n72 = local write "Zolix_USB连接"(FALSE ("温度采集开关")) -> ()
        n73 = call <vilib>:"Add State(s) to Queue__JKI_lib_State_Machine.vi"("State(s) in (\"\")"=w192) -> ("States Out"=w191:string)  [unwired: 14 in]
      }
      frame "---------- UI ----------" {
        # "#CSM \"Category Seperator\"\nDo not put any code in this frame."
        n74 = call <vilib>:"Add State(s) to Queue__JKI_lib_State_Machine.vi"("State(s) in (\"\")"=w195) -> ("States Out"=w194:string)  [unwired: 14 in]
      }
      frame "UI: Initialize" {
        # "#CSM \"Category Seperator\"\nDo not put any code in this frame."
        n75 = Unbundle By Name(w196) -> ("Device Status.运动距离"=w198:dbl, "Device Info.坐标选择"=w200:enum32{"X", "Y", "Z", "T"}, "Device Info.USB Port"=w201:refnum<visa-resource-name>, "Device Info.采集间隔(s)"=w204:dbl, "子程序？"=w203:bool)
        n76 = Not(x=w203) -> (.not. x?=w202:bool)
        n77 = local write "USB Port"(w201) -> ()
        n78 = local write "Interval(s)"(w204) -> ()
        n79 = local write "坐标选择"(w200) -> ()
        n80 = local write "运动距离"(w198) -> ()
        n81 = property on="停止" class="Bool"("Visible"=w202) -> ()  [unwired: 2 in, 2 out]
        n82 = property on="Zolix循环功能" class="Bool (严格)"("DisabledEnum"=T5."Disabled and Grayed Out" ("禁用")) -> ()  [unwired: 2 in, 2 out]
        n83 = property on="Zolix电机位置" class="WFChart (严格)"("History Data"=waveform(dbl)[] [] ("历史数据")) -> ()  [unwired: 2 in, 2 out]
        n84 = call <vilib>:"Add State(s) to Queue__JKI_lib_State_Machine.vi"("State(s) in (\"\")"=w206) -> ("States Out"=w205:string)  [unwired: 14 in]
      }
      frame "UI: Update Graph" {
        # "#CSM \"Category Seperator\"\nDo not put any code in this frame."
        n85 = Unbundle By Name(w215) -> ("Time and Data.Data"=w212:dbl[], "Device Info.采集间隔(s)"=w209:dbl, "Time and Data.采集时间"=w210:timestamp)
        n86 = Index Array(array=w212) -> (element #1=w211:dbl, element #2=w208:dbl)  [unwired: 2 in]
        n87 = Build Array(w211) -> (w214:dbl[])
        n88 = Build Array(w208) -> (w213:dbl[])
        n89 = Bundle By Name("Y"=w214, "t0"=w210, "dt"=w209) -> (→"Zolix电机位置":waveform(dbl))  [unwired: 1 in]
        n90 = Bundle By Name("Y"=w213, "t0"=w210, "dt"=w209) -> ()  [unwired: 1 in, 1 out]
        n91 = call <vilib>:"Add State(s) to Queue__JKI_lib_State_Machine.vi"("State(s) in (\"\")"=w217) -> ("States Out"=w216:string)  [unwired: 14 in]
      }
      frame "---------- Macro ----------" {
        # "#CSM \"Category Seperator\"\nDo not put any code in this frame."
        n92 = call <vilib>:"Add State(s) to Queue__JKI_lib_State_Machine.vi"("State(s) in (\"\")"=w220) -> ("States Out"=w219:string)  [unwired: 14 in]
      }
      frame "Macro: Initialize" {
        w223 = "Data: Initialize\nInitialize Core Data\nUI: Initialize\n\n//Permanent registrations\nAcquired Data@Acquisition - <1> >> Data: Update Indicators -><register>\nAcquired Data@Acquisition - <1> >> API: Log@Logging - <1> -><register>\n\n//Error registrations\nError Occurred@Acquisition - <1> >> Error Handler -><register>\nError Occurred@Logging - <1> >> Error Handler -><register>\n\n//Dynamic registrations\n// 订阅/取消订阅\n//Status@SourceModule >> API@TargetModule -><register as interrupt>\n//UrgentEvent @SourceModule >> API@TargetModule -><register as status>\n\n\n\n//Launch Acquisition Module\n"  # Data: Initialize Initialize Core Data UI: Initialize  //Permanent registrations Acquired Data@Acquisition - <1> >> Data: Update Indicators -><register> Acquired Data@Acquisition - <1> >> API: Log@Logging - <1> -><register>  //Error registrations Error Occurred@Acquisition - <1> >> Error Handler -><register> Error Occurred@Logging - <1> >> Error Handler -><register>  //Dynamic registrations // 订阅/取消订阅 //Status@SourceModule >> API@TargetModule -><register as interrupt> //UrgentEvent @SourceModule >> API@TargetModule -><register as status>    //Launch Acquisition Module
        # "#CSM \"Macro: Initialize\"\nInitialization Macro (This is called once, when the VI starts)"
        n93 = call-poly <userlib>:"Build Message with Arguments++.vi"("States With Replace Token"=w223, "<1>"=w222) -> ("States"=w221:string)  [unwired: 13 in]
        n94 = call <vilib>:"Add State(s) to Queue__JKI_lib_State_Machine.vi"("State(s) in Front (\"\")"=w221, "State(s) in (\"\")"=w226) -> ("States Out"=w225:string)  [unwired: 13 in]
      }
      frame "Macro: Start" {
        n95 = Unbundle By Name(w250) -> ("Device Info.USB Port"=w233:refnum<visa-resource-name>)
        n96 = Unbundle By Name(T6 {"波特率"=19200, "数据位"=8, "校验"=enum."None", "停止位"=10, "流控制"=0} ("串口设置")) -> ("波特率"=w236:u32, "数据位"=w237:u16, "校验"=w238:enum16{"None", "Odd", "Even", "Mark", "Space"}, "停止位"=w239:u16, "流控制"=w240:u16)
        n97 = local write "Zolix_USB连接"(TRUE ("温度采集开关")) -> ()
        n98 = property on="Zolix循环功能" class="Bool (严格)"("DisabledEnum"=T5."Enabled" ("禁用")) -> ()  [unwired: 2 in, 2 out]
        n99 = call-poly "VISA Configure Serial Port"("VISA resource name"=w233, "timeout (10sec)"=u32 3000, "baud rate (9600)"=w236, "data bits (8)"=w237, "parity (0:none)"=w238, "stop bits (10: 1 bit)"=w239, "flow control (0:none)"=w240) -> ("VISA resource name out"=w232:refnum<visa-resource-name>, "error out"=w230:errorcluster)  [unwired: 2 in, 5 out]
        n100 = Bundle By Name(cluster=w250, "Device Info.USB Port"=w232) -> (w242:T11)
        n101 = Unbundle By Name(w242) -> ("Device Info"=w241:T9)
        n102 = call "Fetch.vi"("错误输入"=w230, "Command"="hello", "VISA资源"=w232) -> ("错误输出"=w229:errorcluster, "成功？"=w228:bool)  [unwired: 3 in, 4 out]
        n103 = case shown="True" w228 {
          frame False {
            n104 = local write "状态信息"("USB连接失败!") -> ()
          }
          frame True {
            n105 = local write "状态信息"("USB连接成功！") -> ()
          }
        }
        n106 = call "Convert Data To API String Arguments.vim"("Data"=w241) -> ("API String"=w248:string)  [unwired: 7 in, 1 out]
        n107 = call-poly <userlib>:"Build Message with Arguments++.vi"("States With Replace Token"="API: Start >> <param> -@ Acquisition - <1>\nAPI: Start  -@ Logging - <1>\nAction: Get Unit\nAction: Get Speed" ("State"), "<param>"=w248, "<1>"=w247) -> ("States"=w245:string)  [unwired: 12 in]
        n108 = Select(t=w245, s=w228, f="") -> (s? t:f=w243:string)
        n109 = call <vilib>:"Add State(s) to Queue__JKI_lib_State_Machine.vi"("State(s) in Front (\"\")"=w243, "State(s) in (\"\")"=w252) -> ("States Out"=w251:string)  [unwired: 13 in]
      }
      frame "Macro: Stop" {
        # "#CSM \"Macro: Exit\"\nExit Macro (This is called once, when the VI exits)"
        n110 = call-poly <userlib>:"Build Message with Arguments++.vi"("States With Replace Token"="//Send Message to Other CSM Modules\nAPI: Stop -@ Acquisition - <1>\nAPI: Stop -@ Logging - <1>\n\nMacro: Close", "<1>"=w257) -> ("States"=w256:string)  [unwired: 13 in]
        n111 = call <vilib>:"Add State(s) to Queue__JKI_lib_State_Machine.vi"("State(s) in Front (\"\")"=w256, "State(s) in (\"\")"=w260) -> ("States Out"=w259:string)  [unwired: 13 in]
      }
      frame "Macro: Close" {
        w261 = FALSE ("Zolix_USB连接")
        n112 = Unbundle By Name(w265) -> ("Device Info.USB Port"=w264:refnum<visa-resource-name>)
        n113 = VISA Close(VISA resource name=w264, error in (no error)=w263) -> (error out=w262:errorcluster)
        n114 = local write "Zolix_USB连接"(w261) -> ()
        n115 = local write "Zolix循环功能"(w261) -> ()
        n116 = local write "状态信息"("断开成功!") -> ()
      }
      frame "Macro: Exit" {
        w270 = "//Exit\nMacro: Exit-@Acquisition - <1>\nMacro: Exit-@Logging - <1>\nMacro: Close\n\n\n//Permanent unregistrations\nAcquired Data@Acquisition - <1> >> Data: Update Indicators -><unregister>\nAcquired Data@Acquisition - <1> >> API: Log@Logging - <1> -><unregister>\n\n//Permanent unregistrations\nError Occurred@Acquisition - <1> >> Error Handler -><unregister>\nError Occurred@Logging - <1> >> Error Handler -><unregister>\n\nData: Cleanup\nExit"  # //Exit Macro: Exit-@Acquisition - <1> Macro: Exit-@Logging - <1> Macro: Close   //Permanent unregistrations Acquired Data@Acquisition - <1> >> Data: Update Indicators -><unregister> Acquired Data@Acquisition - <1> >> API: Log@Logging - <1> -><unregister>  //Permanent unregistrations Error Occurred@Acquisition - <1> >> Error Handler -><unregister> Error Occurred@Logging - <1> >> Error Handler -><unregister>  Data: Cleanup Exit
        # "#CSM \"Macro: Exit\"\nExit Macro (This is called once, when the VI exits)"
        n117 = call-poly <userlib>:"Build Message with Arguments++.vi"("States With Replace Token"=w270, "<1>"=w269) -> ("States"=w268:string)  [unwired: 13 in]
        n118 = call <vilib>:"Add State(s) to Queue__JKI_lib_State_Machine.vi"("State(s) in Front (\"\")"=w268, "State(s) in (\"\")"=w273) -> ("States Out"=w272:string)  [unwired: 13 in]
      }
      frame "---------- Action ----------" {
        # "#CSM \"Category Seperator\"\nDo not put any code in this frame."
        n119 = call <vilib>:"Add State(s) to Queue__JKI_lib_State_Machine.vi"("State(s) in (\"\")"=w274) -> ("States Out"=w275:string)  [unwired: 14 in]
      }
      frame "Action: Connect" {
        # "#CSM \"Category Seperator\"\nDo not put any code in this frame."
        n120 = call <vilib>:"Add State(s) to Queue__JKI_lib_State_Machine.vi"("State(s) in (\"\")"=w277) -> ("States Out"=w278:string)  [unwired: 14 in]
      }
      frame "Action: Zolix Stop" {
        # "#CSM \"Category Seperator\"\nDo not put any code in this frame."
        n121 = Unbundle By Name(w287) -> ("Device Info.USB Port"=w286:refnum<visa-resource-name>, "Device Info.Axis"=w284:string[], "Device Info.坐标选择"=w283:enum32{"X", "Y", "Z", "T"})
        n122 = Index Array(array=w284, index=w283) -> (element=w281:string)
        n123 = Concatenate Strings("Stop ", w281) -> (w280:string)
        n124 = call "Fetch.vi"("错误输入"=w285, "Command"=w280, "VISA资源"=w286) -> ()  [unwired: 3 in, 6 out]
        n125 = call <vilib>:"Add State(s) to Queue__JKI_lib_State_Machine.vi"("State(s) in (\"\")"=w288) -> ("States Out"=w289:string)  [unwired: 14 in]
      }
      frame "Action: Axis" {
        # "#CSM \"Category Seperator\"\nDo not put any code in this frame."
        n126 = call "Convert API String Arguments to Data.vim"("Reference Type"=enum32{"X", "Y", "Z", "T"}."X" ("坐标选择"), "API String"=w295) -> ("Data"=w292:enum32{"X", "Y", "Z", "T"})  [unwired: 6 in, 1 out]
        n127 = Bundle By Name(cluster=w293, "Device Info.坐标选择"=w292) -> (w291:T11)
        n128 = call <vilib>:"Add State(s) to Queue__JKI_lib_State_Machine.vi"("State(s) in Front (\"\")"="Action: Get Unit\nAction: Get Speed" ("State(s) in Front (\"\")"), "State(s) in (\"\")"=w296) -> ("States Out"=w297:string)  [unwired: 13 in]
      }
      frame "Action: Change Distance" {
        n129 = call "Convert API String Arguments to Data.vim"("Reference Type"=0.0, "API String"=w302) -> ("Data"=w300:dbl)  [unwired: 6 in, 1 out]
        n130 = local write "运动距离"(w300) -> ()
        n131 = Bundle By Name(cluster=w299, "Device Status.运动距离"=w300) -> (w298:T11)
        n132 = call <vilib>:"Add State(s) to Queue__jki_lib_state_machine.vi"("State(s) in (\"\")"=w303) -> ("States Out"=w304:string)  [unwired: 14 in]
      }
      frame "Action: Set Unit" {
        # "#CSM \"Category Seperator\"\nDo not put any code in this frame."
        n133 = call "Convert API String Arguments to Data.vim"("Reference Type"=Unit."mm" ("单位"), "API String"=w322) -> ("Data"=w307:T1)  [unwired: 6 in, 1 out]
        n134 = Unbundle By Name(w320) -> ("Device Info.USB Port"=w318:refnum<visa-resource-name>, "Device Info.Axis"=w312:string[], "Device Info.坐标选择"=w313:enum32{"X", "Y", "Z", "T"}, "Device Info.Unit"=w310:string[])
        n135 = Index Array(array=w312, index=w313) -> (element=w314:string)
        n136 = Index Array(array=w310, index=w307) -> (element=w309:string)
        n137 = Concatenate Strings("SetUnit ", w314, "," ("字符串"), w309) -> (w308:string)
        n138 = call "Fetch.vi"("错误输入"=w317, "Command"=w308, "VISA资源"=w318) -> ("错误输出"=w316:errorcluster)  [unwired: 3 in, 5 out]
        n139 = Bundle By Name(cluster=w320, "Device Status.单位"=w307) -> (w321:T11)
        n140 = call <vilib>:"Add State(s) to Queue__JKI_lib_State_Machine.vi"("State(s) in Front (\"\")"="Action: Get Unit\nAction: Get Speed" ("State(s) in Front (\"\")"), "State(s) in (\"\")"=w323) -> ("States Out"=w324:string)  [unwired: 13 in]
      }
      frame "Action: Get Unit" {
        # "SetUnit?"
        n141 = Unbundle By Name(w334) -> ("Device Info.USB Port"=w331:refnum<visa-resource-name>, "Device Info.Axis"=w328:string[], "Device Info.坐标选择"=w327:enum32{"X", "Y", "Z", "T"})
        n142 = Index Array(array=w328, index=w327) -> (element=w330:string)
        n143 = Concatenate Strings("SetUnit? ", w330) -> (w326:string)
        n144 = call "Fetch.vi"("Command"=w326, "VISA资源"=w331) -> ("结果字符串"=w325:string)  [unwired: 4 in, 5 out]
        n145 = case shown="\"M\", \"m\", 默认" w325 {
          tunnel: [Unit."deg" ("单位") Unit."mm" ("单位") Unit."PP" ("单位") Unit."um" ("单位")] -> w333
          frame "D", "d" {
          }
          frame "M", "m", Default {
          }
          frame "S", "s" {
          }
          frame "U", "u" {
          }
        }
        n146 = local write "单位"(w333) -> ()
        n147 = Bundle By Name(cluster=w334, "Device Status.单位"=w333) -> (w332:T11)
        n148 = call <vilib>:"Add State(s) to Queue__JKI_lib_State_Machine.vi"("State(s) in (\"\")"=w335) -> ("States Out"=w336:string)  [unwired: 14 in]
      }
      frame "Action: Get Speed" {
        n149 = Unbundle By Name(w365) -> ("Device Info.USB Port"=w362:refnum<visa-resource-name>, "Device Info.Axis"=w361:string[], "Device Info.坐标选择"=w360:enum32{"X", "Y", "Z", "T"})
        n150 = Index Array(array=w361, index=w360) -> (element=w343:string)
        n151 = Concatenate Strings("SetSpeed? ", w343) -> (w364:string)
        n152 = Concatenate Strings("SetAccSpeed? ", w343) -> (w352:string)
        n153 = call "Fetch.vi"("Command"=w364, "VISA资源"=w362) -> ("错误输出"=w356:errorcluster, "数值"=w355:dbl, "VISA资源"=w357:refnum<visa-resource-name>)  [unwired: 4 in, 3 out]
        n154 = local write "常速度"(w355) -> ()
        n155 = Concatenate Strings("SetHomeSpeed? ", w343) -> (w350:string)
        n156 = Concatenate Strings("SetInitSpeed? ", w343) -> (w359:string)
        n157 = call "Fetch.vi"("错误输入"=w356, "Command"=w359, "VISA资源"=w357) -> ("错误输出"=w346:errorcluster, "数值"=w354:dbl, "VISA资源"=w351:refnum<visa-resource-name>)  [unwired: 3 in, 3 out]
        n158 = call "Fetch.vi"("错误输入"=w346, "Command"=w352, "VISA资源"=w351) -> ("错误输出"=w345:errorcluster, "数值"=w344:dbl, "VISA资源"=w348:refnum<visa-resource-name>)  [unwired: 3 in, 3 out]
        n159 = local write "加速度"(w344) -> ()
        n160 = call "Fetch.vi"("错误输入"=w345, "Command"=w350, "VISA资源"=w348) -> ("错误输出"=w342:errorcluster, "数值"=w347:dbl)  [unwired: 3 in, 4 out]
        n161 = local write "归零速度"(w347) -> ()
        n162 = local write "初速度"(w354) -> ()
        n163 = call <vilib>:"Add State(s) to Queue__JKI_lib_State_Machine.vi"("State(s) in (\"\")"=w366) -> ("States Out"=w367:string)  [unwired: 14 in]
      }
      frame "Action: Set Constant Speed" {
        # "SetSpeed axis, speed"
        n164 = Unbundle By Name(w380) -> ("Device Info.USB Port"=w374:refnum<visa-resource-name>, "Device Info.Axis"=w373:string[], "Device Info.坐标选择"=w372:enum32{"X", "Y", "Z", "T"})
        n165 = call "Convert API String Arguments to Data.vim"("Reference Type"=0.0, "API String"=w379) -> ("Data"=w370:dbl)  [unwired: 6 in, 1 out]
        n166 = Number To Fractional String(number=w370) -> (F-format string=w369:string)  [unwired: 3 in]
        n167 = Index Array(array=w373, index=w372) -> (element=w375:string)
        n168 = Concatenate Strings("SetSpeed ", w375, "," ("字符串"), w369) -> (w377:string)
        n169 = call "Fetch.vi"("Command"=w377, "VISA资源"=w374) -> ()  [unwired: 4 in, 6 out]
        n170 = call <vilib>:"Add State(s) to Queue__JKI_lib_State_Machine.vi"("State(s) in Front (\"\")"="Action: Get Speed", "State(s) in (\"\")"=w381) -> ("States Out"=w382:string)  [unwired: 13 in]
      }
      frame "Action: Set Initial Speed" {
        n171 = Unbundle By Name(w386) -> ("Device Info.USB Port"=w392:refnum<visa-resource-name>, "Device Info.Axis"=w391:string[], "Device Info.坐标选择"=w390:enum32{"X", "Y", "Z", "T"})
        n172 = call "Convert API String Arguments to Data.vim"("Reference Type"=0.0, "API String"=w385) -> ("Data"=w388:dbl)  [unwired: 6 in, 1 out]
        n173 = Number To Fractional String(number=w388) -> (F-format string=w387:string)  [unwired: 3 in]
        n174 = Index Array(array=w391, index=w390) -> (element=w393:string)
        n175 = Concatenate Strings("SetInitSpeed ", w393, "," ("字符串"), w387) -> (w395:string)
        n176 = call "Fetch.vi"("Command"=w395, "VISA资源"=w392) -> ()  [unwired: 4 in, 6 out]
        n177 = call <vilib>:"Add State(s) to Queue__JKI_lib_State_Machine.vi"("State(s) in Front (\"\")"="Action: Get Speed", "State(s) in (\"\")"=w397) -> ("States Out"=w398:string)  [unwired: 13 in]
      }
      frame "Action: Set Acc Speed" {
        n178 = Unbundle By Name(w402) -> ("Device Info.USB Port"=w408:refnum<visa-resource-name>, "Device Info.Axis"=w407:string[], "Device Info.坐标选择"=w406:enum32{"X", "Y", "Z", "T"})
        n179 = call "Convert API String Arguments to Data.vim"("Reference Type"=0.0, "API String"=w401) -> ("Data"=w404:dbl)  [unwired: 6 in, 1 out]
        n180 = Number To Fractional String(number=w404) -> (F-format string=w403:string)  [unwired: 3 in]
        n181 = Index Array(array=w407, index=w406) -> (element=w409:string)
        n182 = Concatenate Strings("SetAccSpeed ", w409, "," ("字符串"), w403) -> (w411:string)
        n183 = call "Fetch.vi"("Command"=w411, "VISA资源"=w408) -> ()  [unwired: 4 in, 6 out]
        n184 = call <vilib>:"Add State(s) to Queue__JKI_lib_State_Machine.vi"("State(s) in Front (\"\")"="Action: Get Speed", "State(s) in (\"\")"=w413) -> ("States Out"=w414:string)  [unwired: 13 in]
      }
      frame "Action: Set Home Speed" {
        (unwired) "Action: Get Speed"
        n185 = Unbundle By Name(w418) -> ("Device Info.USB Port"=w424:refnum<visa-resource-name>, "Device Info.Axis"=w423:string[], "Device Info.坐标选择"=w422:enum32{"X", "Y", "Z", "T"})
        n186 = call "Convert API String Arguments to Data.vim"("Reference Type"=0.0, "API String"=w417) -> ("Data"=w420:dbl)  [unwired: 6 in, 1 out]
        n187 = Number To Fractional String(number=w420) -> (F-format string=w419:string)  [unwired: 3 in]
        n188 = Index Array(array=w423, index=w422) -> (element=w425:string)
        n189 = Concatenate Strings("SetHomeSpeed ", w425, "," ("字符串"), w419) -> (w427:string)
        n190 = call "Fetch.vi"("Command"=w427, "VISA资源"=w424) -> ()  [unwired: 4 in, 6 out]
        n191 = call <vilib>:"Add State(s) to Queue__JKI_lib_State_Machine.vi"("State(s) in Front (\"\")"="" ("State(s) in Front (\"\")"), "State(s) in (\"\")"=w429) -> ("States Out"=w430:string)  [unwired: 13 in]
      }
      frame "Action: Absolute Position1" {
        w439 = "," ("字符串")
        # "GoPosition X,O,R,P,5"
        n192 = Unbundle By Name(w449) -> ("Device Info.USB Port"=w443:refnum<visa-resource-name>, "Device Info.Axis"=w442:string[], "Device Info.坐标选择"=w441:enum32{"X", "Y", "Z", "T"})
        n193 = Greater Than 0?(x="位置坐标1") -> (x > 0?=w437:bool)
        n194 = Absolute Value(x="位置坐标1") -> (abs(x)=w433:dbl)
        n195 = Select(t="P", s=w437, f="N") -> (s? t:f=w434:string)
        n196 = Number To Fractional String(number=w433) -> (F-format string=w432:string)  [unwired: 3 in]
        n197 = Index Array(array=w442, index=w441) -> (element=w445:string)
        n198 = Concatenate Strings("GoPosition ", w445, w439, "O" ("字符串"), w439, "A" ("字符串"), w439, w434, w439, w432) -> (w446:string)
        n199 = call "Fetch.vi"("Command"=w446, "VISA资源"=w443) -> ()  [unwired: 4 in, 6 out]
        n200 = call <vilib>:"Add State(s) to Queue__JKI_lib_State_Machine.vi"("State(s) in (\"\")"=w447) -> ("States Out"=w448:string)  [unwired: 14 in]
      }
      frame "Action: Absolute Position2" {
        w462 = "," ("字符串")
        n201 = Unbundle By Name(w454) -> ("Device Info.USB Port"=w466:refnum<visa-resource-name>, "Device Info.Axis"=w465:string[], "Device Info.坐标选择"=w464:enum32{"X", "Y", "Z", "T"})
        n202 = Greater Than 0?(x="位置坐标2") -> (x > 0?=w460:bool)
        n203 = Absolute Value(x="位置坐标2") -> (abs(x)=w456:dbl)
        n204 = Select(t="P", s=w460, f="N") -> (s? t:f=w457:string)
        n205 = Number To Fractional String(number=w456) -> (F-format string=w455:string)  [unwired: 3 in]
        n206 = Index Array(array=w465, index=w464) -> (element=w468:string)
        n207 = Concatenate Strings("GoPosition ", w468, w462, "O" ("字符串"), w462, "A" ("字符串"), w462, w457, w462, w455) -> (w469:string)
        n208 = call "Fetch.vi"("Command"=w469, "VISA资源"=w466) -> ("错误输出"=w452:errorcluster)  [unwired: 4 in, 5 out]
        n209 = flat-sequence {
          tunnel: [w474] -> w470
          tunnel: w452 -> [w474]
          frame #0 {
            n210 = Wait (ms)(milliseconds to wait=u32 30 ("等待时间（毫秒）")) -> ()  [unwired: 1 out]
          }
        }
        n211 = call <vilib>:"Add State(s) to Queue__JKI_lib_State_Machine.vi"("State(s) in (\"\")"=w471) -> ("States Out"=w472:string)  [unwired: 14 in]
      }
      frame "Action: Move" {
        w485 = "," ("字符串")
        # "GoPosition X,O,R,P,5"
        # "后退 下0\n前进 上1"
        n212 = call "Convert API String Arguments to Data.vim"("Reference Type"=u32 0 ("floor(x/y)"), "API String"=w494) -> ("Data"=w477:u32)  [unwired: 6 in, 1 out]
        n213 = Greater Than 0?(x=w477) -> (x > 0?=w483:bool)
        n214 = Unbundle By Name(w478) -> ("Device Info.USB Port"=w489:refnum<visa-resource-name>, "Device Info.Axis"=w488:string[], "Device Info.坐标选择"=w487:enum32{"X", "Y", "Z", "T"}, "Device Status.运动距离"=w475:dbl)
        n215 = Select(t="P", s=w483, f="N") -> (s? t:f=w480:string)
        n216 = Absolute Value(x=w475) -> (abs(x)=w476:dbl)
        n217 = Index Array(array=w488, index=w487) -> (element=w491:string)
        n218 = Number To Fractional String(number=w476) -> (F-format string=w479:string)  [unwired: 3 in]
        n219 = Concatenate Strings("GoPosition ", w491, w485, "O" ("字符串"), w485, "R" ("字符串"), w485, w480, w485, w479) -> (w492:string)
        n220 = call "Fetch.vi"("Command"=w492, "VISA资源"=w489) -> ()  [unwired: 4 in, 6 out]
        n221 = call <vilib>:"Add State(s) to Queue__JKI_lib_State_Machine.vi"("State(s) in (\"\")"=w495) -> ("States Out"=w496:string)  [unwired: 14 in]
      }
      frame "Action: Continuous Move" {
        n222 = call "Convert API String Arguments to Data.vim"("Reference Type"=u32 0 ("floor(x/y)"), "API String"=w498) -> ("Data"=w500:u32)  [unwired: 6 in, 1 out]
        n223 = Greater Than 0?(x=w500) -> (x > 0?=w504:bool)
        n224 = Unbundle By Name(w499) -> ("Device Info.USB Port"=w508:refnum<visa-resource-name>, "Device Info.Axis"=w507:string[], "Device Info.坐标选择"=w506:enum32{"X", "Y", "Z", "T"})
        n225 = Select(t="P", s=w504, f="N") -> (s? t:f=w501:string)
        n226 = Index Array(array=w507, index=w506) -> (element=w510:string)
        n227 = Concatenate Strings("Go ", w510, "," ("字符串"), w501) -> (w511:string)
        n228 = call "Fetch.vi"("Command"=w511, "VISA资源"=w508) -> ()  [unwired: 4 in, 6 out]
        n229 = call <vilib>:"Add State(s) to Queue__JKI_lib_State_Machine.vi"("State(s) in (\"\")"=w513) -> ("States Out"=w514:string)  [unwired: 14 in]
      }
      frame "Action: Negative Limit Zero" {
        n230 = Unbundle By Name(w529) -> ("Device Info.USB Port"=w525:refnum<visa-resource-name>, "Device Info.Axis"=w524:string[], "Device Info.坐标选择"=w523:enum32{"X", "Y", "Z", "T"})
        n231 = Index Array(array=w524, index=w523) -> (element=w517:string)
        n232 = Concatenate Strings("Setsechhomemode ", w517, "," ("字符串"), "1" ("字符串")) -> (w528:string)
        n233 = call "Fetch.vi"("Command"=w528, "VISA资源"=w525) -> ("错误输出"=w520:errorcluster, "VISA资源"=w521:refnum<visa-resource-name>)  [unwired: 4 in, 4 out]
        n234 = Concatenate Strings("GoHome " ("字符串"), w517) -> (w516:string)
        n235 = call "Fetch.vi"("错误输入"=w520, "Command"=w516, "VISA资源"=w521) -> ("错误输出"=w519:errorcluster)  [unwired: 3 in, 5 out]
        n236 = call <vilib>:"Add State(s) to Queue__JKI_lib_State_Machine.vi"("State(s) in (\"\")"=w530) -> ("States Out"=w531:string)  [unwired: 14 in]
      }
      frame "Action: Optical Zero" {
        n237 = Unbundle By Name(w532) -> ("Device Info.USB Port"=w541:refnum<visa-resource-name>, "Device Info.Axis"=w540:string[], "Device Info.坐标选择"=w539:enum32{"X", "Y", "Z", "T"})
        n238 = Index Array(array=w540, index=w539) -> (element=w534:string)
        n239 = Concatenate Strings("Setsechhomemode ", w534, "," ("字符串"), "2" ("字符串")) -> (w544:string)
        n240 = call "Fetch.vi"("Command"=w544, "VISA资源"=w541) -> ("错误输出"=w536:errorcluster, "VISA资源"=w537:refnum<visa-resource-name>)  [unwired: 4 in, 4 out]
        n241 = Concatenate Strings("GoHome " ("字符串"), w534) -> (w533:string)
        n242 = call "Fetch.vi"("错误输入"=w536, "Command"=w533, "VISA资源"=w537) -> ()  [unwired: 3 in, 6 out]
        n243 = call <vilib>:"Add State(s) to Queue__JKI_lib_State_Machine.vi"("State(s) in (\"\")"=w545) -> ("States Out"=w546:string)  [unwired: 14 in]
      }
      frame "Action: User Zero" {
        n244 = Unbundle By Name(w548) -> ("Device Info.USB Port"=w557:refnum<visa-resource-name>, "Device Info.Axis"=w556:string[], "Device Info.坐标选择"=w555:enum32{"X", "Y", "Z", "T"})
        n245 = Index Array(array=w556, index=w555) -> (element=w550:string)
        n246 = Concatenate Strings("SetOrigin ", w550, "," ("字符串"), "2" ("字符串")) -> (w560:string)
        n247 = call "Fetch.vi"("Command"=w560, "VISA资源"=w557) -> ("错误输出"=w552:errorcluster, "VISA资源"=w553:refnum<visa-resource-name>)  [unwired: 4 in, 4 out]
        n248 = Concatenate Strings("GoOrigin " ("字符串"), w550) -> (w549:string)
        n249 = call "Fetch.vi"("错误输入"=w552, "Command"=w549, "VISA资源"=w553) -> ()  [unwired: 3 in, 6 out]
        n250 = call <vilib>:"Add State(s) to Queue__JKI_lib_State_Machine.vi"("State(s) in (\"\")"=w561) -> ("States Out"=w562:string)  [unwired: 14 in]
      }
      frame "---------- API ----------" {
        # "#CSM \"Category Seperator\"\nDo not put any code in this frame."
        n251 = call <vilib>:"Add State(s) to Queue__JKI_lib_State_Machine.vi"("State(s) in (\"\")"=w564) -> ("States Out"=w565:string)  [unwired: 14 in]
      }
      frame "API: Sample Interval" {
        # "#CSM \"Category Seperator\"\nDo not put any code in this frame."
        n252 = call-poly <userlib>:"Build Message with Arguments++.vi"("States With Replace Token"="API: Sample Interval >> <param> ->| Acquisition - <1>" ("State"), "<param>"=w569, "<1>"=w573) -> ("States"=w572:string)  [unwired: 12 in]
        n253 = call "Convert API String Arguments to Data.vim"("Reference Type"=0.5 ("Interval(s)"), "API String"=w569) -> ("Data"=w570:dbl)  [unwired: 6 in, 1 out]
        n254 = Bundle By Name(cluster=w568, "Device Info.采集间隔(s)"=w570) -> (w567:T11)
        n255 = call <vilib>:"Add State(s) to Queue__JKI_lib_State_Machine.vi"("State(s) in Front (\"\")"=w572, "State(s) in (\"\")"=w575) -> ("States Out"=w576:string)  [unwired: 13 in]
      }
      frame "API: USB Port" {
        # "#CSM \"Category Seperator\"\nDo not put any code in this frame."
        n256 = call "Convert API String Arguments to Data.vim"("Reference Type"=refnum<visa-resource-name> refnum ("USB Port"), "API String"=w580) -> ("Data"=w581:refnum<visa-resource-name>)  [unwired: 6 in, 1 out]
        n257 = Bundle By Name(cluster=w579, "Device Info.USB Port"=w581) -> (w578:T11)
        n258 = call <vilib>:"Add State(s) to Queue__JKI_lib_State_Machine.vi"("State(s) in (\"\")"=w582) -> ("States Out"=w583:string)  [unwired: 14 in]
      }
      frame "---------- Repeat ----------" {
        n259 = call <vilib>:"Add State(s) to Queue__JKI_lib_State_Machine.vi"("State(s) in (\"\")"=w584) -> ("States Out"=w585:string)  [unwired: 14 in]
      }
      frame "Repeat: Enable" {
        w592 = T13 [{"行程"=25.0, "时间(s)"=60.0, "进度"=1.000390362739563, "光谱测量拿起"=FALSE, "运行方向"=FALSE, "速度"=25.0, "分段颜色"=enum."蓝色"}, {"行程"=26.0, "时间(s)"=60.0, "进度"=1.0013926823933919, "光谱测量拿起"=TRUE, "运行方向"=FALSE, "速度"=25.0, "分段颜色"=enum."蓝色"}, {"行程"=25.0, "时间(s)"=60.0, "进度"=1.0006222248077392, "光谱测量拿起"=FALSE, "运行方向"=FALSE, "速度"=25.0, "分段颜色"=enum."蓝色"}, {"行程"=26.0, "时间(s)"=60.0, "进度"=0.6612281163533529, "光谱测量拿起"=TRUE, "运行方向"=FALSE, "速度"=25.0, "分段颜色"=enum."蓝色"}]  # 循环步骤
        n260 = call "CSM - Read Configuration Variable.vim"("Section Name (\"\" as Default)"=w590, "Configuration Prototype (Cluster Prefered)"=w592) -> ("Configuration"=w597:T13)  [unwired: 6 in, 1 out]
        n261 = control-ref of="子面板-Repeat"() -> (w588:refnum<vi>)
        n262 = Concatenate Strings("Repeat - " ("Name(\"\" to use uuid)"), w590) -> (w594:string)
        n263 = vi-ref "UI-Zolix.lvlib:Repeat.lvlib:Repeat.vi"() -> (w593:refnum<vi>)
        n264 = call "Convert Data To API String Arguments.vim"("Data"=w597) -> ("API String"=w596:string)  [unwired: 7 in, 1 out]
        n265 = flat-sequence {
          tunnel: [w607] -> w589
          tunnel: w590 -> [w605]
          tunnel: w595 -> [_]
          tunnel: w596 -> [w602]
          frame #0 {
            w609 = "Error Occurred@Repeat - <1> >> Error Handler -><register>\nRepeat Changed@Repeat - <1> >> Save Repeat -><register>"  # Error Occurred@Repeat - <1> >> Error Handler -><register> Repeat Changed@Repeat - <1> >> Save Repeat -><register>
            n266 = Wait (ms)(milliseconds to wait=u32 100 ("等待时间（毫秒）")) -> ()  [unwired: 1 out]
            n267 = call <vilib>:"Add State(s) to Queue__JKI_lib_State_Machine.vi"("State(s) in Front (\"\")"=w609, "State(s) in (\"\")"="API: CSM Name  >> <1> ->| Repeat - <1> ", "State(s) at Back (\"\")"="API: INI Read  >> <param> ->| Repeat - <1> ") -> ("States Out"=w608:string)  [unwired: 12 in]
            n268 = call-poly <userlib>:"Build Message with Arguments++.vi"("States With Replace Token"=w608, "<param>"=w602, "<1>"=w605) -> ("States"=w607:string)  [unwired: 12 in]
          }
        }
        n269 = call "打开引用.vi"("引用"=w588, "CSM Name"=w594, "VI"=w593) -> ("错误输出"=w595:errorcluster)  [unwired: 7 in, 1 out]
        n270 = call <vilib>:"Add State(s) to Queue__JKI_lib_State_Machine.vi"("State(s) in Front (\"\")"=w589, "State(s) in (\"\")"=w598) -> ("States Out"=w599:string)  [unwired: 13 in]
      }
      frame "Save Repeat" {
        w613 = T13 [{"行程"=25.0, "时间(s)"=60.0, "进度"=1.000390362739563, "光谱测量拿起"=FALSE, "运行方向"=FALSE, "速度"=25.0, "分段颜色"=enum."蓝色"}, {"行程"=26.0, "时间(s)"=60.0, "进度"=1.0013926823933919, "光谱测量拿起"=TRUE, "运行方向"=FALSE, "速度"=25.0, "分段颜色"=enum."蓝色"}, {"行程"=25.0, "时间(s)"=60.0, "进度"=1.0006222248077392, "光谱测量拿起"=FALSE, "运行方向"=FALSE, "速度"=25.0, "分段颜色"=enum."蓝色"}, {"行程"=26.0, "时间(s)"=60.0, "进度"=0.6612281163533529, "光谱测量拿起"=TRUE, "运行方向"=FALSE, "速度"=25.0, "分段颜色"=enum."蓝色"}]  # 循环步骤
        # "save\n结束后控件自动变F"
        n271 = call "Convert API String Arguments to Data.vim"("Reference Type"=w613, "API String"=w611) -> ("Data"=w612:T13)  [unwired: 6 in, 1 out]
        n272 = call "CSM - Write Configuration Variable.vim"("Section Name (\"\" as Default)"=w610, "Configuration"=w612) -> ()  [unwired: 6 in, 2 out]
        n273 = call <vilib>:"Add State(s) to Queue__JKI_lib_State_Machine.vi"("State(s) in (\"\")"=w614) -> ("States Out"=w615:string)  [unwired: 14 in]
      }
      frame "Repeat: Disable" {
        w622 = "Error Occurred@Repeat - <1> >> Error Handler -><unregister>\nRepeat Changed@Repeat - <1> >> Save Repeat -><unregister>"  # Error Occurred@Repeat - <1> >> Error Handler -><unregister> Repeat Changed@Repeat - <1> >> Save Repeat -><unregister>
        n274 = call <vilib>:"Add State(s) to Queue__JKI_lib_State_Machine.vi"("State(s) in Front (\"\")"=w622, "State(s) in (\"\")"="Macro: Exit-@Repeat - <1>", "State(s) at Back (\"\")"="Repeat: Remove" ("State(s) at Back (\"\")")) -> ("States Out"=w620:string)  [unwired: 12 in]
        n275 = call-poly <userlib>:"Build Message with Arguments++.vi"("States With Replace Token"=w620) -> ("States"=w618:string)  [unwired: 14 in]
        n276 = call <vilib>:"Add State(s) to Queue__JKI_lib_State_Machine.vi"("State(s) in Front (\"\")"=w618, "State(s) in (\"\")"=w623) -> ("States Out"=w624:string)  [unwired: 13 in]
      }
      frame "Repeat: Remove" {
        n277 = control-ref of="子面板-Repeat"() -> (w627:refnum<vi>)
        n278 = invoke class="SubPnl" method="Remove VI"(reference=w627) -> (error out=w628:errorcluster)  [unwired: 2 in, 2 out]
        n279 = vi-ref "UI-Zolix.lvlib:Repeat.lvlib:Repeat.vi"() -> (w629:refnum<vi>)
        n280 = call "关闭引用.vi"("错误输入（无错误）"=w628, "引用"=w629) -> ()  [unwired: 9 in, 1 out]
        n281 = call <vilib>:"Add State(s) to Queue__JKI_lib_State_Machine.vi"("State(s) in (\"\")"=w630) -> ("States Out"=w631:string)  [unwired: 14 in]
      }
    }
    n282 = Unbundle By Name(w26) -> ("子程序？"=w25:bool)
    n283 = call "State Delete.vi"("Delete?(F)"=w25, "CSM name to delete"=string[] ["Logging"], "State In"=w29) -> ("State Out"=w28:string)  [unwired: 8 in]
  }
  n284 = while {
    shift-right: [w644] -> _
    shift-left: enum16{"Idle", "Initialize", "Exit"}."Initialize" -> [w645]
    tunnel: "CSM Name" -> [w642]
    shift-right: [w640] -> _
    shift-left: w9 -> [w641]
    shift-right: [w638] -> _
    shift-left: -1 -> [w639]
    shift-right: [w637] -> _
    shift-left: _ -> [w636]
    shift-right: [w635] -> _
    shift-left: _ -> [w634]
    stop <- w643 stop-if-true
    n285 = case shown="\"Idle\", 默认" w645 {
      tunnel: [enum16{"Idle", "Initialize", "Exit"}."Idle" w663 enum16{"Idle", "Initialize", "Exit"}."Exit"] -> w644
      tunnel: [_ _ TRUE] -> w643
      tunnel: w642 -> [w649 w662 _]
      tunnel: w641 -> [w652 w660 w829]
      tunnel: [w652 w661 w829] -> w640
      tunnel: w639 -> [_ w658 _]
      tunnel: [-1 w659 _] -> w638
      tunnel: [w648 w656 _] -> w637
      tunnel: w636 -> [_ w657 w828]
      tunnel: [w646 w654 w826] -> w635
      tunnel: w634 -> [_ w655 w826]
      frame "Initialize" {
        w647 = FALSE  # your data
        n286 = call <userlib>:"CSM - Module Exit Event.vi"("Name (\"\" to Use UUID) In"=w649) -> ("CSM Exit Event"=w650:refnum<user-event>)  [unwired: 8 in, 2 out]
        n287 = register-events(w650) -> (reference out=w648:refnum<event-registration>)  [unwired: 2 in, 1 out]
        n288 = Bundle("your data"=w647) -> (w646:cluster{"your data":bool})  [unwired: 1 in]
      }
      frame "Idle", Default {
        n289 = event shown="[13] \"位置1\": 值改变" {
          selector: w657 -> [_ _ _ _ _ _ _ _ _ _ _ _ _ _ _ _ _ _ _ _ _ _ _]
          dyn-events: [_ _ _ _ _ _ _ _ _ _ _ _ _ _ _ _ _ _ _ _ _ _ _] -> w656
          timeout: w658 -> [_ _ _ _ _ _ _ _ _ _ _ _ _ _ _ _ _ _ _ _ _ _ _]
          tunnel: [_ w670 enum16{"Idle", "Initialize", "Exit"}."Exit" _ _ _ _ _ _ _ _ _ _ _ _ _ _ _ _ _ _ _ _] -> w663
          tunnel: w662 -> [w665 w675 _ _ _ _ _ _ _ _ _ _ _ _ _ _ _ _ _ _ _ _ _]
          tunnel: w660 -> [w668 _ w685 w691 w700 w703 w710 w717 w724 w731 w738 w745 w752 w756 w760 w772 w784 w788 w792 w796 w801 w808 w814]
          tunnel: [w666 w674 w685 w692 w699 w704 w711 w718 w725 w732 w739 w746 w753 w757 w761 w773 w785 w789 w793 w797 w800 w807 w815] -> w661
          tunnel: [-1 _ _ _ _ _ _ _ _ _ _ _ _ _ _ _ _ _ _ _ _ _ _] -> w659
          tunnel: w655 -> [w664 w673 w683 w693 w701 w705 w712 w719 w726 w733 w740 w747 w754 w758 w762 w774 w786 w790 w794 w798 w805 w812 w820]
          tunnel: [w664 w673 w683 w693 w701 w705 w712 w719 w726 w733 w740 w747 w754 w758 w762 w774 w786 w790 w794 w798 w805 w812 w820] -> w654
          event Timeout {
            n290 = event-data() -> ()  [unwired: 1 in, 3 out]
            n291 = call-poly <userlib>:"CSM - Filter JKISM String Queue.vi"("States In"=w668) -> ("States Out"=w667:string)  [unwired: 14 in]
            n292 = call <userlib>:"CSM - Forward UI Operations to CSM.vi"("Name (\"\" to Use UUID)"=w665, "State(s) In (\"\")"=w667) -> ("States Out"=w666:string)  [unwired: 8 in, 1 out]
          }
          event Panel Close? {
            n293 = event-data() -> ()  [unwired: 1 in, 1 out]
            n294 = Two Button Dialog(message="确定关闭程序？" ("消息")) -> (T button?=w671:bool)  [unwired: 2 in]
            n295 = case shown="False" w671 {
              tunnel: w675 -> [w678 w681]
              tunnel: [w678 w680] -> w674
              tunnel: [enum16{"Idle", "Initialize", "Exit"}."Idle" enum16{"Idle", "Initialize", "Exit"}."Exit"] -> w670
              frame False {
              }
              frame True {
                n296 = call <userlib>:"CSM - Forward UI Operations to CSM.vi"("Name (\"\" to Use UUID)"=w681, "State(s) In (\"\")"="Macro: Exit" ("State")) -> ("States Out"=w680:string)  [unwired: 8 in, 1 out]
              }
            }
            n297 = event-data("Discard?"=TRUE) -> ()  [unwired: 1 in, 1 out]
          }
          event User Event {
            n298 = event-data() -> ()  [unwired: 1 in, 1 out]
          }
          event "停止": Value Change {
            n299 = event-data() -> ()  [unwired: 1 in, 1 out]
            n300 = Two Button Dialog(message="确定停止程序？" ("消息")) -> (T button?=w688:bool)  [unwired: 2 in]
            n301 = Select(t="Macro: Exit" ("State(s) in Front (\"\")"), s=w688, f="") -> (s? t:f=w686:string)
            n302 = call <vilib>:"Add State(s) to Queue__JKI_lib_State_Machine.vi"("State(s) in Front (\"\")"=w686, "State(s) in (\"\")"=w691) -> ("States Out"=w692:string)  [unwired: 13 in]
          }
          event "Zolix_USB连接": Value Change {
            n303 = event-data() -> ()  [unwired: 1 in, 1 out]
            n304 = Select(t="Macro: Start" ("State(s) in Front (\"\")"), s="Zolix_USB连接", f="Macro: Stop" ("State(s) in Front (\"\")")) -> (s? t:f=w696:string)
            n305 = local write "Error Occurred"(errorcluster {"status"=FALSE, "code"=0, "source"=""} ("错误常量")) -> ()
            n306 = call <vilib>:"Add State(s) to Queue__JKI_lib_State_Machine.vi"("State(s) in Front (\"\")"=w696, "State(s) in (\"\")"=w700) -> ("States Out"=w699:string)  [unwired: 13 in]
          }
          event "Zolix停止": Value Change {
            n307 = event-data() -> ()  [unwired: 1 in, 1 out]
            n308 = call <vilib>:"Add State(s) to Queue__JKI_lib_State_Machine.vi"("State(s) in Front (\"\")"="Action: Zolix Stop", "State(s) in (\"\")"=w703) -> ("States Out"=w704:string)  [unwired: 13 in]
          }
          event "坐标选择": Value Change {
            n309 = event-data() -> ()  [unwired: 1 in, 1 out]
            n310 = call "Convert Data To API String Arguments.vim"("Data"="坐标选择") -> ("API String"=w709:string)  [unwired: 7 in, 1 out]
            n311 = call <vilib>:"Build State String with Arguments__JKI_lib_State_Machine.vi"("Arguments (\"\")"=w709, "State"="Action: Axis") -> ("State with Arguments"=w707:string)  [unwired: 4 in]
            n312 = call <vilib>:"Add State(s) to Queue__JKI_lib_State_Machine.vi"("State(s) in Front (\"\")"=w707, "State(s) in (\"\")"=w710) -> ("States Out"=w711:string)  [unwired: 13 in]
          }
          event "运动距离": Value Change {
            n313 = event-data() -> ()  [unwired: 1 in, 1 out]
            n314 = call "Convert Data To API String Arguments.vim"("Data"="运动距离") -> ("API String"=w716:string)  [unwired: 7 in, 1 out]
            n315 = call <vilib>:"Build State String with Arguments__JKI_lib_State_Machine.vi"("Arguments (\"\")"=w716, "State"="Action: Change Distance") -> ("State with Arguments"=w714:string)  [unwired: 4 in]
            n316 = call <vilib>:"Add State(s) to Queue__jki_lib_state_machine.vi"("State(s) in Front (\"\")"=w714, "State(s) in (\"\")"=w717) -> ("States Out"=w718:string)  [unwired: 13 in]
          }
          event "常速度": Value Change {
            n317 = event-data() -> ()  [unwired: 1 in, 1 out]
            n318 = call "Convert Data To API String Arguments.vim"("Data"="常速度") -> ("API String"=w723:string)  [unwired: 7 in, 1 out]
            n319 = call <vilib>:"Build State String with Arguments__JKI_lib_State_Machine.vi"("Arguments (\"\")"=w723, "State"="Action: Set Constant Speed") -> ("State with Arguments"=w721:string)  [unwired: 4 in]
            n320 = call <vilib>:"Add State(s) to Queue__JKI_lib_State_Machine.vi"("State(s) in Front (\"\")"=w721, "State(s) in (\"\")"=w724) -> ("States Out"=w725:string)  [unwired: 13 in]
          }
          event "初速度": Value Change {
            n321 = event-data() -> ()  [unwired: 1 in, 1 out]
            n322 = call "Convert Data To API String Arguments.vim"("Data"="初速度") -> ("API String"=w730:string)  [unwired: 7 in, 1 out]
            n323 = call <vilib>:"Build State String with Arguments__JKI_lib_State_Machine.vi"("Arguments (\"\")"=w730, "State"="Action: Set Initial Speed") -> ("State with Arguments"=w728:string)  [unwired: 4 in]
            n324 = call <vilib>:"Add State(s) to Queue__JKI_lib_State_Machine.vi"("State(s) in Front (\"\")"=w728, "State(s) in (\"\")"=w731) -> ("States Out"=w732:string)  [unwired: 13 in]
          }
          event "加速度": Value Change {
            n325 = event-data() -> ()  [unwired: 1 in, 1 out]
            n326 = call "Convert Data To API String Arguments.vim"("Data"="加速度") -> ("API String"=w737:string)  [unwired: 7 in, 1 out]
            n327 = call <vilib>:"Build State String with Arguments__JKI_lib_State_Machine.vi"("Arguments (\"\")"=w737, "State"="Action: Set Acc Speed") -> ("State with Arguments"=w735:string)  [unwired: 4 in]
            n328 = call <vilib>:"Add State(s) to Queue__JKI_lib_State_Machine.vi"("State(s) in Front (\"\")"=w735, "State(s) in (\"\")"=w738) -> ("States Out"=w739:string)  [unwired: 13 in]
          }
          event "归零速度": Value Change {
            n329 = event-data() -> ()  [unwired: 1 in, 1 out]
            n330 = call "Convert Data To API String Arguments.vim"("Data"="归零速度") -> ("API String"=w744:string)  [unwired: 7 in, 1 out]
            n331 = call <vilib>:"Build State String with Arguments__JKI_lib_State_Machine.vi"("Arguments (\"\")"=w744, "State"="Action: Set Home Speed") -> ("State with Arguments"=w742:string)  [unwired: 4 in]
            n332 = call <vilib>:"Add State(s) to Queue__JKI_lib_State_Machine.vi"("State(s) in Front (\"\")"=w742, "State(s) in (\"\")"=w745) -> ("States Out"=w746:string)  [unwired: 13 in]
          }
          event Value Change {
            n333 = event-data() -> ()  [unwired: 1 in, 1 out]
            n334 = call "Convert Data To API String Arguments.vim"("Data"="单位") -> ("API String"=w751:string)  [unwired: 7 in, 1 out]
            n335 = call <vilib>:"Build State String with Arguments__JKI_lib_State_Machine.vi"("Arguments (\"\")"=w751, "State"="Action: Set Unit") -> ("State with Arguments"=w749:string)  [unwired: 4 in]
            n336 = call <vilib>:"Add State(s) to Queue__JKI_lib_State_Machine.vi"("State(s) in Front (\"\")"=w749, "State(s) in (\"\")"=w752) -> ("States Out"=w753:string)  [unwired: 13 in]
          }
          event "位置1": Value Change {
            n337 = event-data() -> ()  [unwired: 1 in, 1 out]
            n338 = call <vilib>:"Add State(s) to Queue__JKI_lib_State_Machine.vi"("State(s) in Front (\"\")"="Action: Absolute Position1", "State(s) in (\"\")"=w756) -> ("States Out"=w757:string)  [unwired: 13 in]
          }
          event "位置2": Value Change {
            n339 = event-data() -> ()  [unwired: 1 in, 1 out]
            n340 = call <vilib>:"Add State(s) to Queue__JKI_lib_State_Machine.vi"("State(s) in Front (\"\")"="Action: Absolute Position2", "State(s) in (\"\")"=w760) -> ("States Out"=w761:string)  [unwired: 13 in]
          }
          event "前进", "后退": Value Change {
            n341 = event-data() -> ()  [unwired: 1 in, 1 out]
            n342 = Build Array("后退", "前进") -> (w770:bool[])
            n343 = Boolean Array To Number(Boolean array=w770) -> (number=w769:u32)
            n344 = Quotient & Remainder(x=w769, y=u32 2) -> (floor(x/y)=w766:u32)  [unwired: 1 out]
            n345 = call "Convert Data To API String Arguments.vim"("Data"=w766) -> ("API String"=w767:string)  [unwired: 7 in, 1 out]
            n346 = call <vilib>:"Build State String with Arguments__JKI_lib_State_Machine.vi"("Arguments (\"\")"=w767, "State"="Action: Move") -> ("State with Arguments"=w764:string)  [unwired: 4 in]
            n347 = call <vilib>:"Add State(s) to Queue__JKI_lib_State_Machine.vi"("State(s) in Front (\"\")"=w764, "State(s) in (\"\")"=w772) -> ("States Out"=w773:string)  [unwired: 13 in]
          }
          event "连续前进", "连续后退": Value Change {
            n348 = event-data() -> ()  [unwired: 1 in, 1 out]
            n349 = Build Array("连续后退", "连续前进") -> (w783:bool[])
            n350 = Boolean Array To Number(Boolean array=w783) -> (number=w782:u32)
            n351 = Quotient & Remainder(x=w782, y=u32 2) -> (floor(x/y)=w779:u32)  [unwired: 1 out]
            n352 = call "Convert Data To API String Arguments.vim"("Data"=w779) -> ("API String"=w780:string)  [unwired: 7 in, 1 out]
            n353 = call <vilib>:"Build State String with Arguments__JKI_lib_State_Machine.vi"("Arguments (\"\")"=w780, "State"="Action: Continuous Move") -> ("State with Arguments"=w775:string)  [unwired: 4 in]
            n354 = call <vilib>:"Add State(s) to Queue__JKI_lib_State_Machine.vi"("State(s) in Front (\"\")"=w775, "State(s) in (\"\")"=w784) -> ("States Out"=w785:string)  [unwired: 13 in]
          }
          event "负限位归零": Value Change {
            n355 = event-data() -> ()  [unwired: 1 in, 1 out]
            n356 = call <vilib>:"Add State(s) to Queue__JKI_lib_State_Machine.vi"("State(s) in Front (\"\")"="Action: Negative Limit Zero", "State(s) in (\"\")"=w788) -> ("States Out"=w789:string)  [unwired: 13 in]
          }
          event "光学归零": Value Change {
            n357 = event-data() -> ()  [unwired: 1 in, 1 out]
            n358 = call <vilib>:"Add State(s) to Queue__JKI_lib_State_Machine.vi"("State(s) in Front (\"\")"="Action: Optical Zero", "State(s) in (\"\")"=w792) -> ("States Out"=w793:string)  [unwired: 13 in]
          }
          event "用户原点归零": Value Change {
            n359 = event-data() -> ()  [unwired: 1 in, 1 out]
            n360 = call <vilib>:"Add State(s) to Queue__JKI_lib_State_Machine.vi"("State(s) in Front (\"\")"="Action: User Zero", "State(s) in (\"\")"=w796) -> ("States Out"=w797:string)  [unwired: 13 in]
          }
          event "Interval(s)": Value Change {
            n361 = event-data() -> ()  [unwired: 1 in, 1 out]
            n362 = call "Convert Data To API String Arguments.vim"("Data"="Interval(s)") -> ("API String"=w803:string)  [unwired: 7 in, 1 out]
            n363 = call <vilib>:"Build State String with Arguments__JKI_lib_State_Machine.vi"("Arguments (\"\")"=w803, "State"="API: Sample Interval" ("State(s) in Front (\"\")")) -> ("State with Arguments"=w802:string)  [unwired: 4 in]
            n364 = call <vilib>:"Add State(s) to Queue__JKI_lib_State_Machine.vi"("State(s) in Front (\"\")"=w802, "State(s) in (\"\")"=w801) -> ("States Out"=w800:string)  [unwired: 13 in]
          }
          event "USB Port": Value Change {
            n365 = event-data() -> ()  [unwired: 1 in, 1 out]
            n366 = call "Convert Data To API String Arguments.vim"("Data"="USB Port") -> ("API String"=w810:string)  [unwired: 7 in, 1 out]
            n367 = call <vilib>:"Build State String with Arguments__JKI_lib_State_Machine.vi"("Arguments (\"\")"=w810, "State"="API: USB Port" ("State(s) in Front (\"\")")) -> ("State with Arguments"=w809:string)  [unwired: 4 in]
            n368 = call <vilib>:"Add State(s) to Queue__JKI_lib_State_Machine.vi"("State(s) in Front (\"\")"=w809, "State(s) in (\"\")"=w808) -> ("States Out"=w807:string)  [unwired: 13 in]
          }
          event "Zolix循环功能": Value Change {
            n369 = event-data() -> ("OldVal"=w817:bool, "NewVal"=w816:bool)  [unwired: 1 in]
            n370 = Not Equal?(x=w817, y=w816) -> (x != y?=w819:bool)
            n371 = case shown="True" w819 {
              tunnel: ["" w823] -> w813
              tunnel: "Zolix循环功能" -> [_ w822]
              frame False {
              }
              frame True {
                n372 = Select(t="Repeat: Enable", s=w822, f="Repeat: Disable") -> (s? t:f=w823:string)
              }
            }
            n373 = call <vilib>:"Add State(s) to Queue__JKI_lib_State_Machine.vi"("State(s) in Front (\"\")"=w813, "State(s) in (\"\")"=w814) -> ("States Out"=w815:string)  [unwired: 13 in]
          }
        }
      }
      frame "Exit" {
        n374 = Unregister For Events(event registration refnum=w828) -> (error out=w827:errorcluster)  [unwired: 1 in]
        n375 = call <vilib>:"Clear Errors.vi"("error in (no error)"=w827) -> ()  [unwired: 5 in, 2 out]
      }
    }
  }
  n376 = flat-sequence {
    tunnel: w5 -> [_]
    tunnel: "CSM Name" -> [w834]
    tunnel: "子程序？" -> [w832]
    frame #0 {
      n377 = Concatenate Strings("Acquisition - " ("Name(\"\" to use uuid)"), w834) -> (w836:string)
      n378 = call "Acquisition.vi"("CSM Name"=w836) -> ()  [unwired: 11 in]
      n379 = Concatenate Strings("Logging - " ("Name(\"\" to use uuid)"), w834) -> (w833:string)
      n380 = case shown="False" w832 {
        tunnel: w833 -> [w838 _]
        frame False {
          n381 = call "Logging.vi"("CSM Name"=w838) -> ()  [unwired: 11 in]
        }
        frame True {
        }
      }
    }
  }
  n382 = call <userlib>:"CSM - Sync Configuration Variables to File.vi"("All Temp Variable to Default Ini(F)"=TRUE, "error in (no error)"=w3) -> ()  [unwired: 7 in, 1 out]
